vi "4Pi Capture Manager.vi"(7 "Calling VI Ref":refnum<vi>) -> ()   [LabVIEW 2021]
uses:
  4Pi Capture Manager Controls/4Pi Capture Switch Laser.ctl
  4Pi Capture Manager Controls/4Pi Capture Switch Line Scan Modes.ctl
  4Pi Capture Manager Controls/4Pi Capture Line Scan Settings.ctl
  4Pi Capture Manager Controls/DM scan mode.ctl
  4Pi Capture Manager Controls/4Pi Capture Acq Settings.ctl
  <vilib>/Utility/miscctls.llb/LVPointTypeDef.ctl
  4Pi Capture Manager Controls/4Pi Capture Notifier Type.ctl
  4Pi Capture Manager Controls/4Pi Capture Actions.ctl
  4Pi Dual DM Control/4Pi Dual DM - Controls/4Pi Dual DM - Mirror Modes.ctl
  <vilib>/vision/Image Controls.llb/IMAQ Image.ctl
  Hardware Configuration/Hardware Configuration Controls/Device Type.ctl
  4Pi Dual DM Control/4Pi Dual DM - Controls/4Pi Dual DM - Standard Action.ctl
  Hardware Configuration/Hardware Configuration Controls/Device Function.ctl
  Device Library/Cameras/Hamamatsu/Orca Flash/Orca Flash Controls/Orca Flash Actions.ctl
  Device Library/Cameras/Hamamatsu/Orca Flash/Orca Flash Controls/Orca Flash Parameters.ctl
  Device Library/Cameras/Hamamatsu/Orca Flash/Orca Flash Controls/Orca Flash Parameter List.ctl
  Device Library/Cameras/Hamamatsu/Orca Flash/Orca Flash Controls/Orca Flash ROI.ctl
  4Pi Capture Manager Controls/4Pi Capture Scan Tracker.ctl
  Device Manager/Common Device Queue/Common Device Controls/Common Device Actions.ctl
  Device Library/Cameras/Hamamatsu/Orca Flash/Orca Flash Controls/Orca Flash Notifier Element.ctl
  Device Library/DAQmx/AO Single Channel Triggered Ramp/AO SCTR Type Defs/AO SCTR Actions.ctl
  Wide Field Drift Correction/WFDC Controls/WFDC External Sync.ctl
  Wide Field Drift Correction/WFDC Controls/WFDC Cycle Pause.ctl
  Wide Field Drift Correction/WFDC Controls/WFDC Status.ctl
  Device Library/Stages/Stages Controls/Stage Actions.ctl
  Device Library/Shutters/Shutter Controls/Shutter Actions.ctl
  Device Library/AOTFs/AOTF Controls/AOTF Actions.ctl
  Device Library/Cameras/Camera Controls/Camera IMAQ Key Info.ctl
  <vilib>/Utility/file.llb/Read Delimited Spreadsheet (DBL).vi
  <vilib>/Utility/file.llb/Write Delimited Spreadsheet (DBL).vi
  shell32.dll
panel:
  in  "Main Tab":T1(tab)
  in  "Sampling Time (s)":dbl min=0.0 format="%#_2f"
  out "Frame":u32(slide) scale=0.0..10.0
  out "Cycle":sgl(slide) scale=0.0..1.0
  in  "Base Save Path":path
  in  "Capture":bool
  in  "Live Preview":bool
  out "Z Step":sgl(slide) scale=0.0..1.0
  in  "File Name":string="Test Image"
  in  "Preview Exposure Time (s)":dbl=0.1 caption="Exposure Time (s)"
  in  "Capture Exposure Time (s)":dbl=0.1 caption="Exposure Time (s)"
  in  "No. of Frames":u32=1 min=1
  in  "No. of Cycles":u16=1 min=1
  in  "No. of Z Steps":u16=1 min=1
  in  "Z Step Size (µm)":dbl min=-10.0 max=10.0
  in  "Switch Laser At":T2=enum."Each Cycle"
  out "Current Cycle":u16
  out "Current Step":u16
  out "Current Frame":u32
  in  "Auto Update Subfolder":bool=TRUE
  in  "Subfolder Name":string="Area"
  in  "Current Laser":u16(ring) items=["560", "642", "405", "488", "940"]
  in  "Save As Preset":bool
  in  "Line Scan Active":bool
  in  "Number of Lines":u32=8 min=1 max=200 step=1
  in  "Line Scan Mode":T3
  in  "Line Scanning Presets":u16(ring) items=["01 FPS", "02 FPS", "04 FPS", "08 FPS", "16 FPS", "40 FPS"]
  in  "Line Scan Settings":T4
  in  "Active option":enum32{"option 1", "option 2", "option 3"}(radio)
  in  "bead collection":bool
  in  "Soft trigger":bool
  in  "DM first":bool
  in  "Amp magnitude":dbl
  in  "DM scan mode":T5 items=["Idle", "Orthogonal", "Random"]
  in  "Amp step size":dbl
  in  "No. Amp steps":u16=1 min=1
  in  "Mirror Mode":u16[](array[numeric])=[1] min=1 max=140
  in  "Camera Settings":bool
  in  "Quadrants On/Off":bool
  in  "Auto Shutter":bool
  in  "acq settings":T6
  in  "Quit":bool
  # "Live Preview"
  # "Capture"
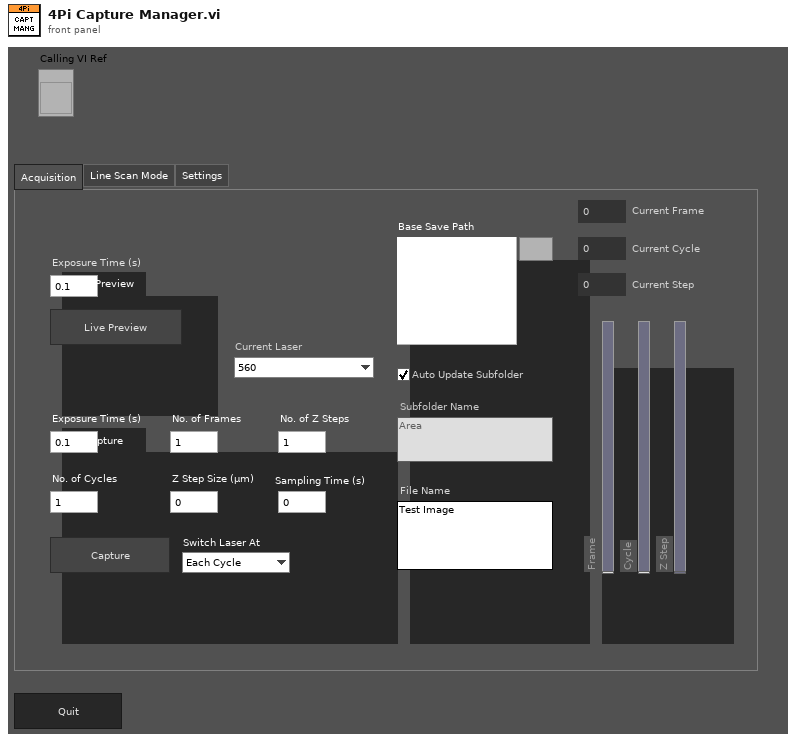
[diagram p1: front panel]
types:
  T1 = enum32{"Acquisition", "Line Scan Mode", "Settings"}
  T2 = typedef "4Pi Capture Switch Laser.ctl" = enum16{"Each Step", "Each Cycle", "All Cycles"}
  T3 = typedef "4Pi Capture Switch Line Scan Modes.ctl" = enum32{"Automatic", "Use Presets", "Manual"}
  T4 = typedef "4Pi Capture Line Scan Settings.ctl" = cluster{"Interline Interval":dbl, "Offset (V)":dbl, "Amplitude (V)":dbl, "Samples Per Channel":dbl, "Delay (ms)":dbl}
  T5 = typedef "DM scan mode.ctl" = u16
  T6 = typedef "4Pi Capture Acq Settings.ctl" = cluster{"Exposure Time (s)":dbl, "No. of Frames":u32, "No. of Z Steps":u16, "No. of Cycles":u16, "Z Step Size (µm)":dbl}
  T7 = typedef "4Pi Dual DM - Standard Action.ctl" = enum16{"Read", "Write"}
  T8 = typedef "IMAQ Image.ctl" = refnum<image>
  T9 = cluster{"Image Ref":T8, "Cycle Number":u16, "Camera Running?":bool, "Capture?":bool}
  T10 = enum8{"Enabled", "Disabled", "Disabled and Grayed Out"}
  T11 = typedef "Device Type.ctl" = enum16{"AOTF", "Camera", "Deformable Mirror", "Laser", "Flip Mirror", "Shutter", "Stage", "Waveform", "FPGA", "Filter Wheel", "Email"}
  T12 = typedef "4Pi Capture Notifier Type.ctl" = cluster{"Actions":T13, "Running?":bool, "Preview Exposure (s)":dbl, "Capture Exposure (s)":dbl, "Cycles":u16, "Frames":u32, "No. of Z Steps":u16, "Z Step Size (µm)":dbl, "Base Path":path, "Init Z Position (µm)":dbl, "Lasers Lines":string[], "Save Path":path, "Line Scan?":bool, "Line Scan Mode":T3, "No. Amp steps":u16, "Amp step size":dbl, "No. Mirror Mode":u16, "DM scan mode":T5, "Metadata File Ref":refnum<file>[], "Init Mirror Modes":T14, "Sampling Time (s)":dbl}
  T13 = typedef "4Pi Capture Actions.ctl" = enum16{"Idle", "Live Preview", "Capture", "Laser On", "Laser Off", "Open Shutters", "Close Shutters", "Set Exposure Time", "Start Acquisition", "Update SubFolder", "Setup", "Camera Soft Trigger", "Camera", "Swtich1", "Switch", "Step", "Cycle", "Write DM", "External Cycle Sync", "Write Metadata", "Abort", "Quit"}
  T14 = typedef "4Pi Dual DM - Mirror Modes.ctl" = cluster{"Mode":string, "Amplitude":dbl}[]
  T15 = enum16{"Always On", "Always Off", "Off While Running"}
  T16 = typedef "LVPointTypeDef.ctl" = cluster{"Horizontal":i16, "Vertical":i16}
  T17 = typedef "Image Type" = u32
  T18 = typedef "Device Function.ctl" = enum16{"Primary", "Secondary", "Overview", "Wide Field Drift Correction", "642 nm Excitation", "560 nm Excitation", "940 nm Excitation", "546 nm Excitation", "488 nm Excitation", "405 nm Excitation", "Objective Drift Correction", "4Pi Focus Lock", "4Pi Objective Lock", "Objective XY", "Objective Z", "Sample XY", "Sample Coarse Z", "Sample Z", "4Pi Lower", "4Pi Upper", "Em Small", "Em Large", "Ex Small", "Ex Large", "Mojo", "Adj Cavity", "Line Scanning", "Alert"}
  T19 = typedef "Orca Flash Parameters.ctl" = cluster{"Value":dbl, "Orca Flash Parameters":T20}
  T20 = typedef "Orca Flash Parameter List.ctl" = u32
  T21 = enum32{"Page Enabled", "Page Disabled", "Page Disabled & Grayed"}
  T22 = typedef "Orca Flash ROI.ctl" = cluster{"H Offset":i32, "V Offset":i32, "H Width":i32, "V Width":i32}
  T23 = typedef "Orca Flash Actions.ctl" = enum16{"IDLE", "PREVIEW", "RECORD", "Send Trigger", "SOFT TRIGGER", "Record Settings", "SETPARAM", "GETPARAM", "SETROI", "GETROI", "PROGRESSIVE MODE", "AREA MODE", "STATUS", "QUIT"}
  T24 = typedef "4Pi Capture Scan Tracker.ctl" = cluster{"Current Step":u16, "Current Cycle":u16, "Current Laser":u16, "# of Lasers":u16, "# of Cycles":u16, "# of Steps":u16, "Switch Laser At":T2, "Current Mirror Mode":u16, "# of Mirror Mode":u16, "Current Amp step":u16, "# of Amp steps":u16}
  T25 = typedef "WFDC Status.ctl" = enum16{"Idle", "Busy", "DC Active", "Error", "Canceled"}
  T26 = typedef "WFDC External Sync.ctl" = cluster{"Cycle Sync":T27, "Z Offset":dbl, "WFDC Status":T25}
  T27 = typedef "WFDC Cycle Pause.ctl" = enum16{"Pause Requested", "Paused", "Resume Requested", "Resumed"}
  T28 = typedef "Stage Actions.ctl" = enum16{"Get Position", "SERVO OFF", "SERVO ON", "SERVO ON/OFF", "MVR", "MOVE", "HALT", "ONTARGET", "ERROR", "REFERENCE", "INIT", "VELOCITY", "STATUS", "EXIT", "HOME", "ZEROPOS", "NANOPOS", "ANALOG", "QUIT"}
  T29 = typedef "Shutter Actions.ctl" = enum16{"Open", "Close", "Toggle", "Status", "Quit"}
  T30 = typedef "AOTF Actions.ctl" = enum16{"Error Check", "Blank", "Line On/Off", "Set Power", "Status", "Quit"}
  T31 = typedef "AO SCTR Actions.ctl" = enum16{"Stop at Offset", "Update and Run", "Quit"}
  T32 = enum16{"open", "replace", "create", "open or create", "replace or create", "replace or create with confirmation"}
  T33 = typedef "Camera IMAQ Key Info.ctl" = cluster{"Frame":u32, "Sensor Height":i32, "Sensor Width":i32, "ROI Height":i32, "ROI Width":i32, "ROI Enable?":bool, "Bit per Pixel":u8}
  T34 = typedef "Orca Flash Notifier Element.ctl" = cluster{"Camera Actions":T23, "Received?":bool, "Running?":bool, "sCMOS Parameter":T19, "sCMOS ROI":T22, "Save Path":path, "# of frames":u32, "Image Ref":T8, "Trigger?":bool, "bead collection":bool}
  T35 = typedef "Common Device Actions.ctl" = enum16{"Specific Action", "Open Front Panel", "Close Front Panel", "Quit", "Quit All"}
  T36 = typedef "4Pi Dual DM - Mirror Modes DUAL.ctl" = cluster{"Mode":string, "Amplitude":dbl}[][]
  T37 = typedef "LVRectTypeDef.ctl" = cluster{"Left":i16, "Top":i16, "Right":i16, "Bottom":i16}
  T38 = typedef "LVBoundsTypeDef.ctl" = cluster{"Width":u32, "Height":u32}
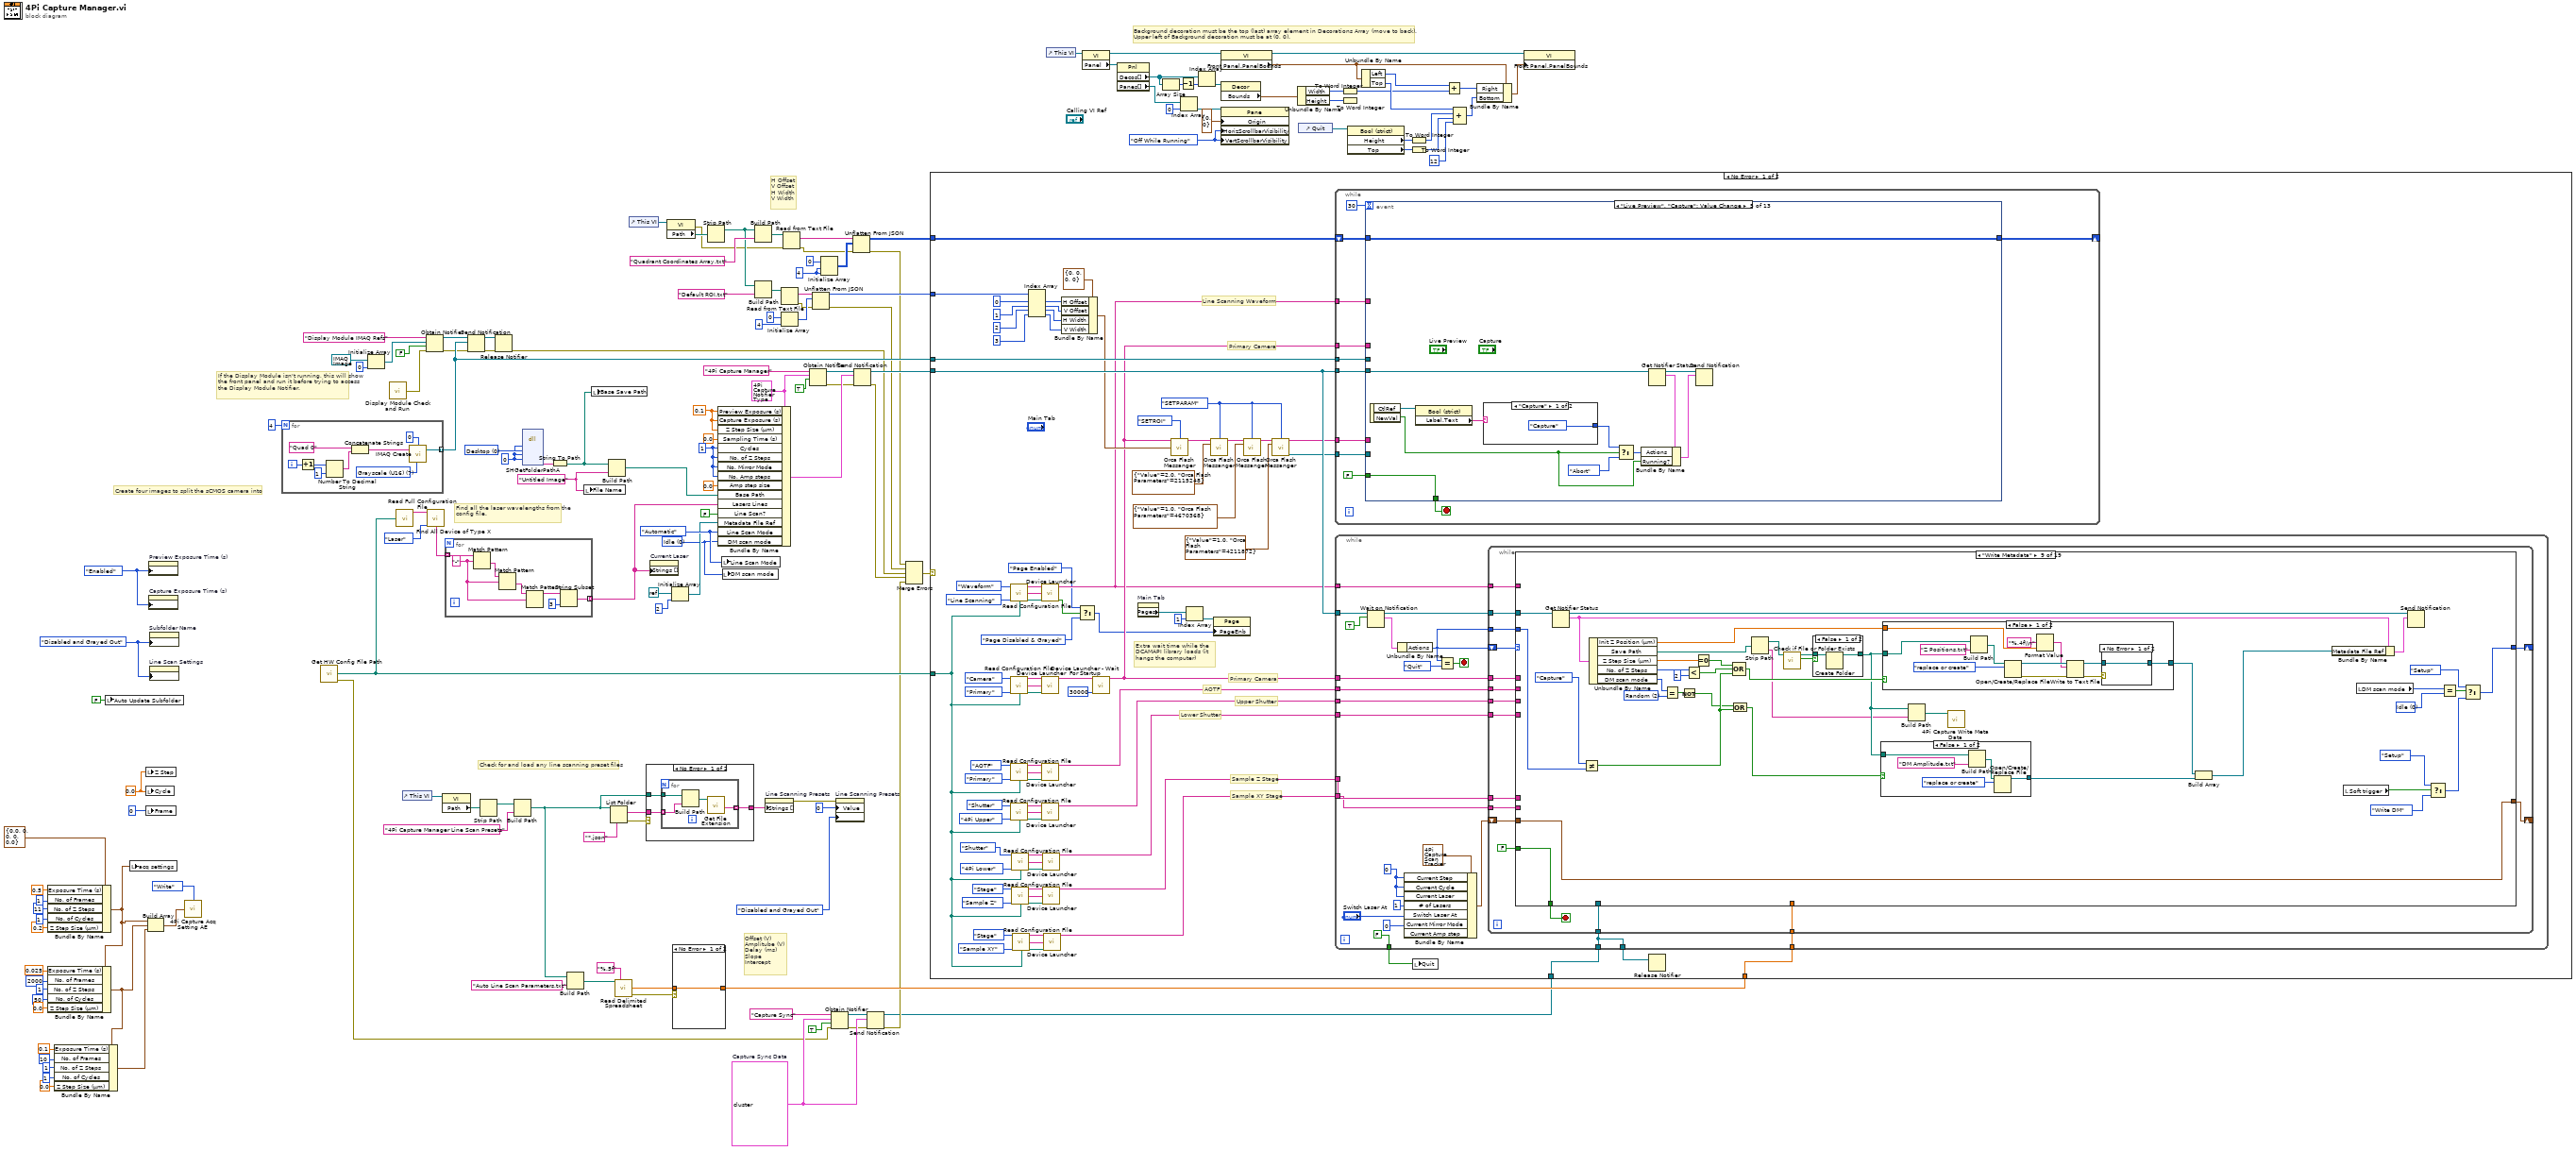
[diagram p0: block diagram]
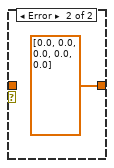
[diagram p2: hidden frame]
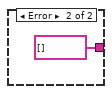
[diagram p3: hidden frame]
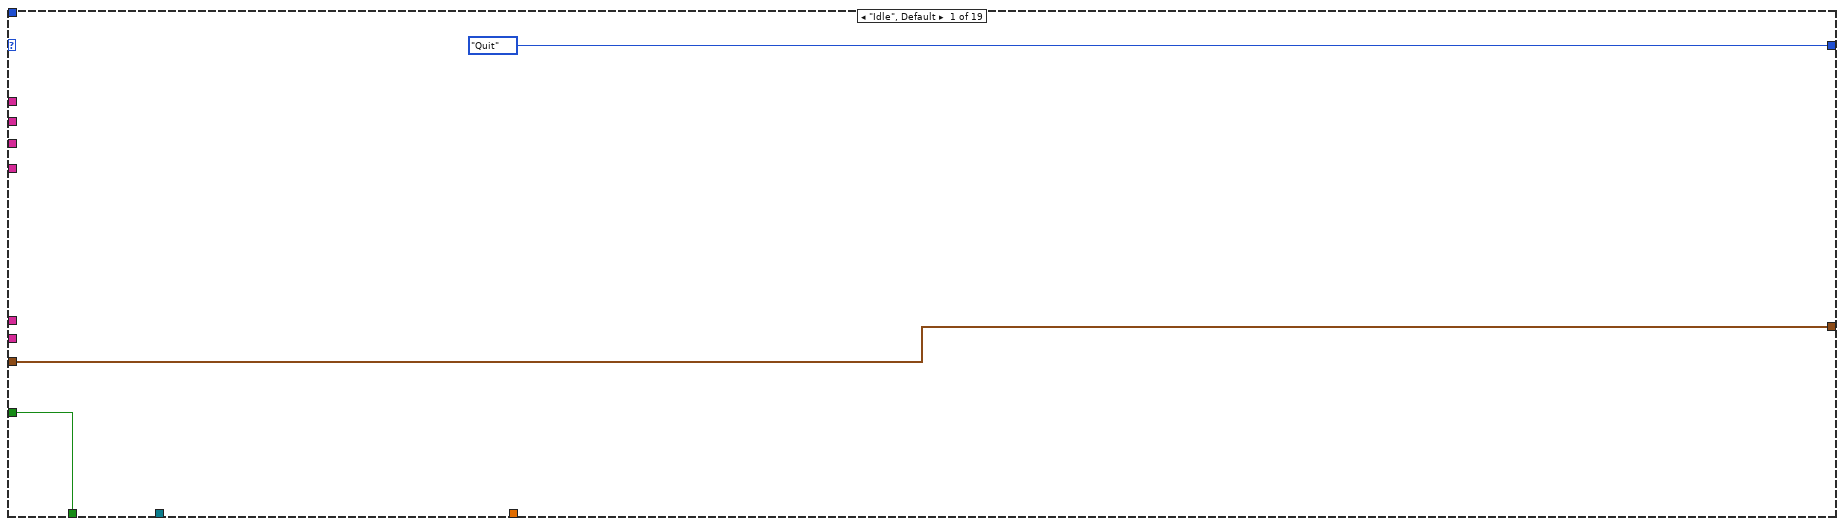
[diagram p4: hidden frame]
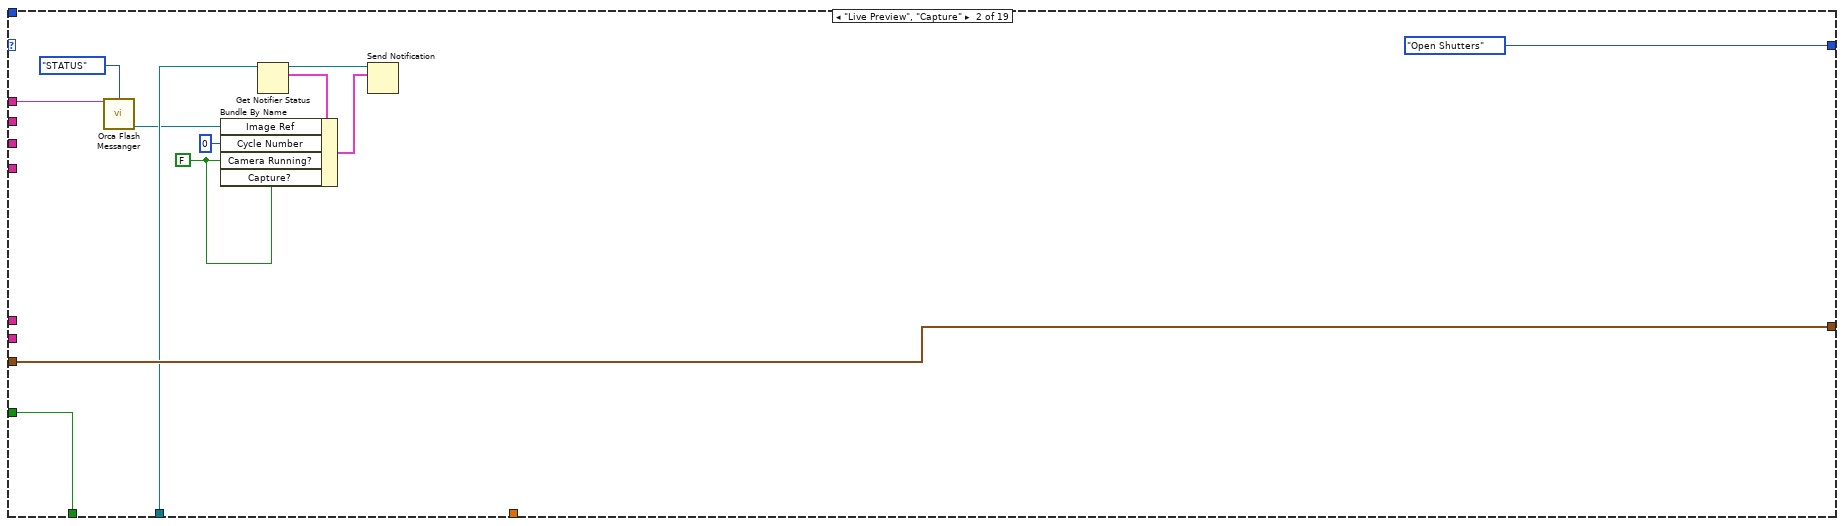
[diagram p5: hidden frame]
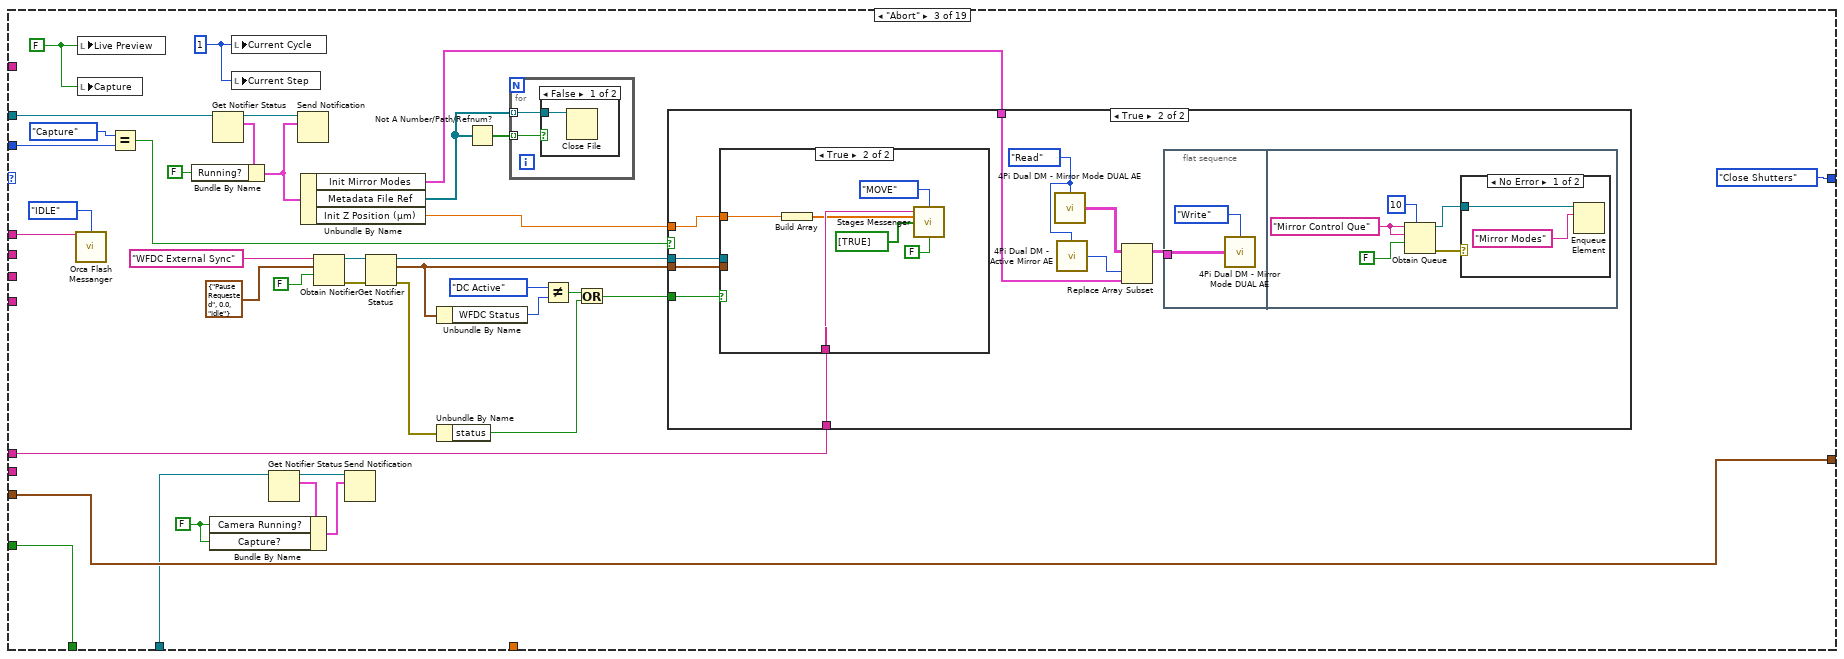
[diagram p6: hidden frame]
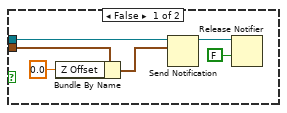
[diagram p10: hidden frame]
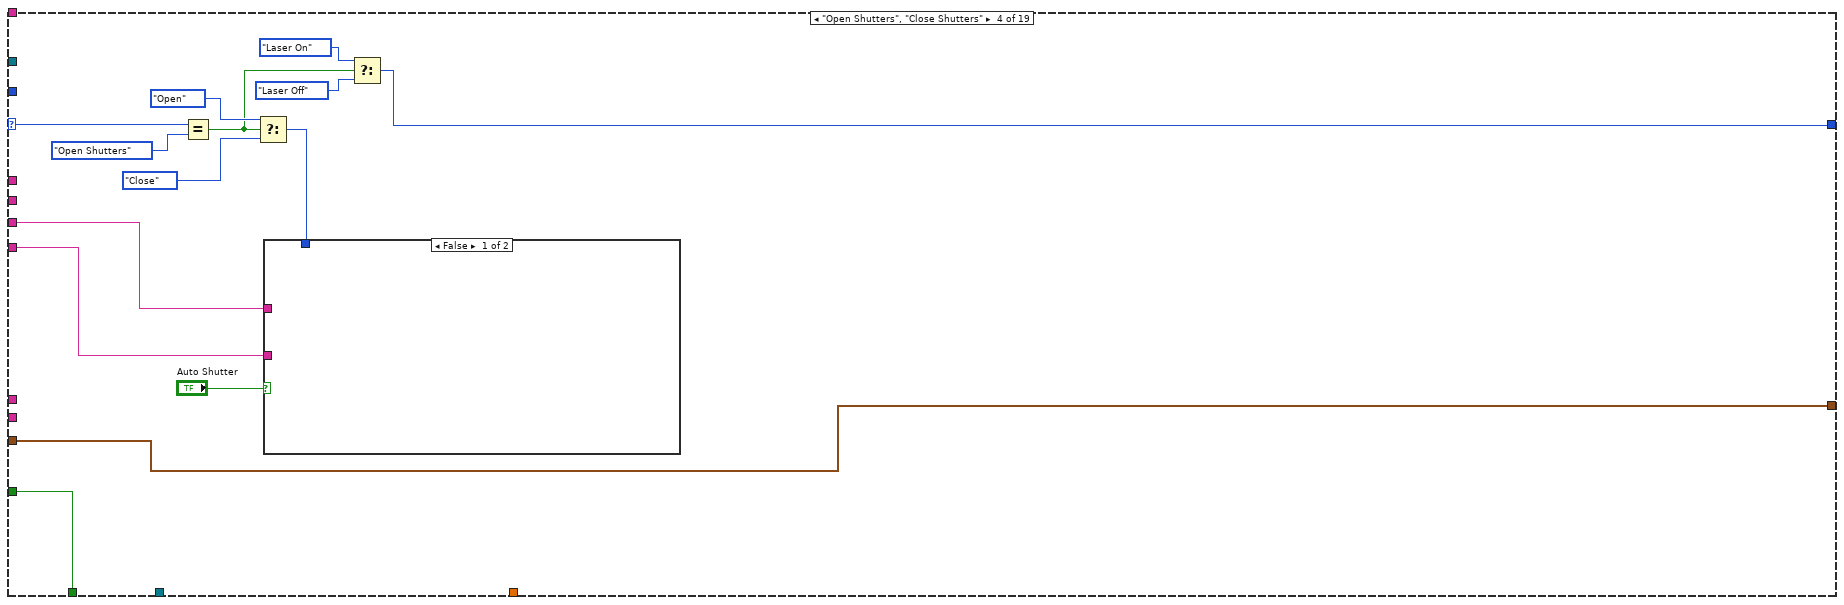
[diagram p11: hidden frame]
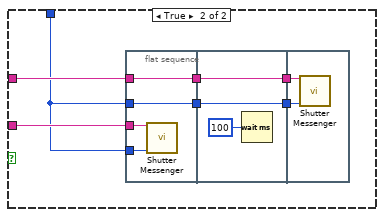
[diagram p12: hidden frame]
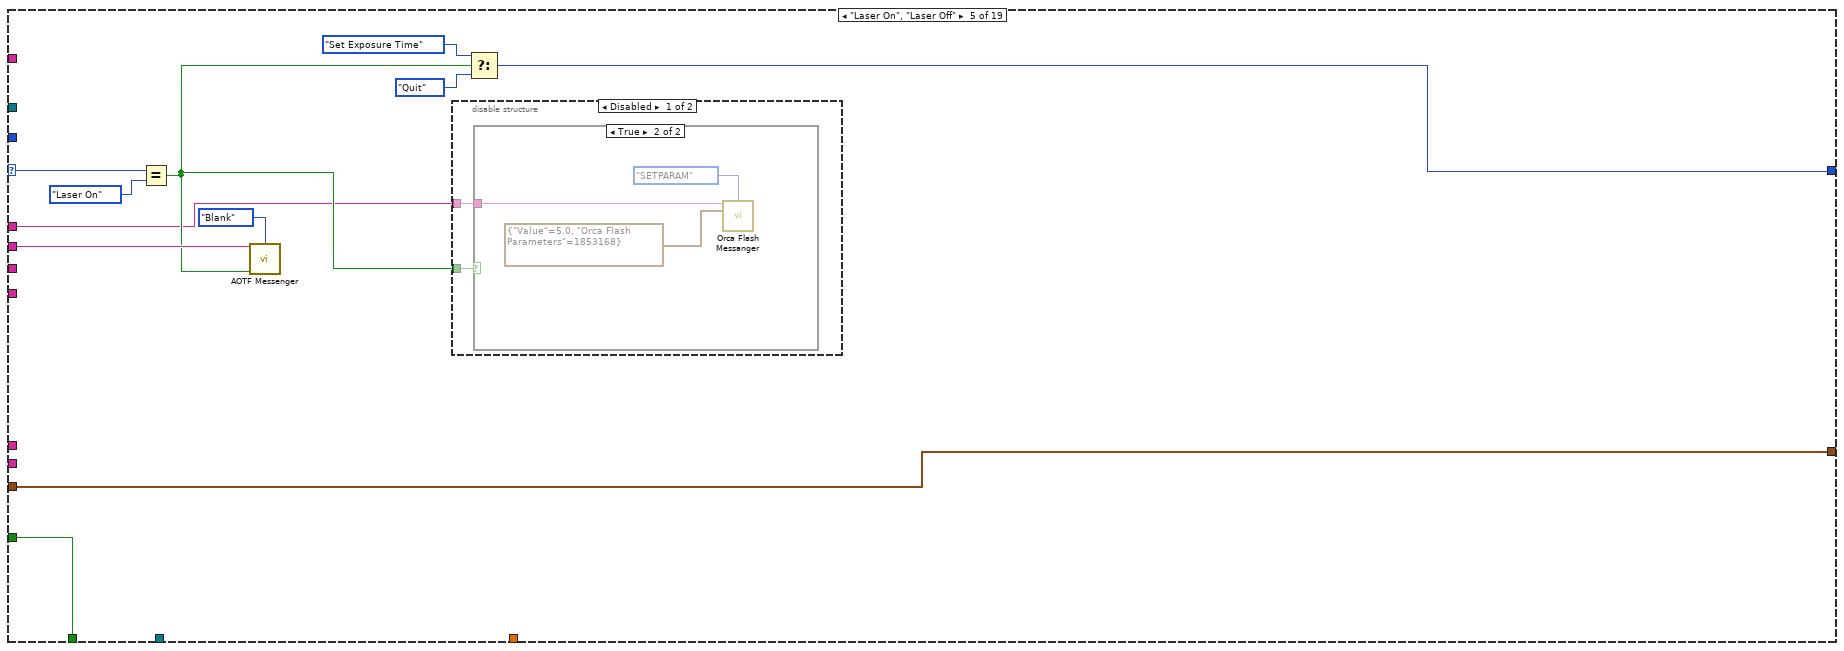
[diagram p13: hidden frame]
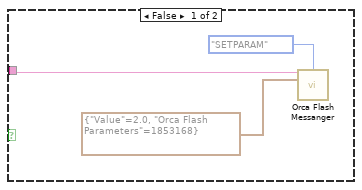
[diagram p14: hidden frame]
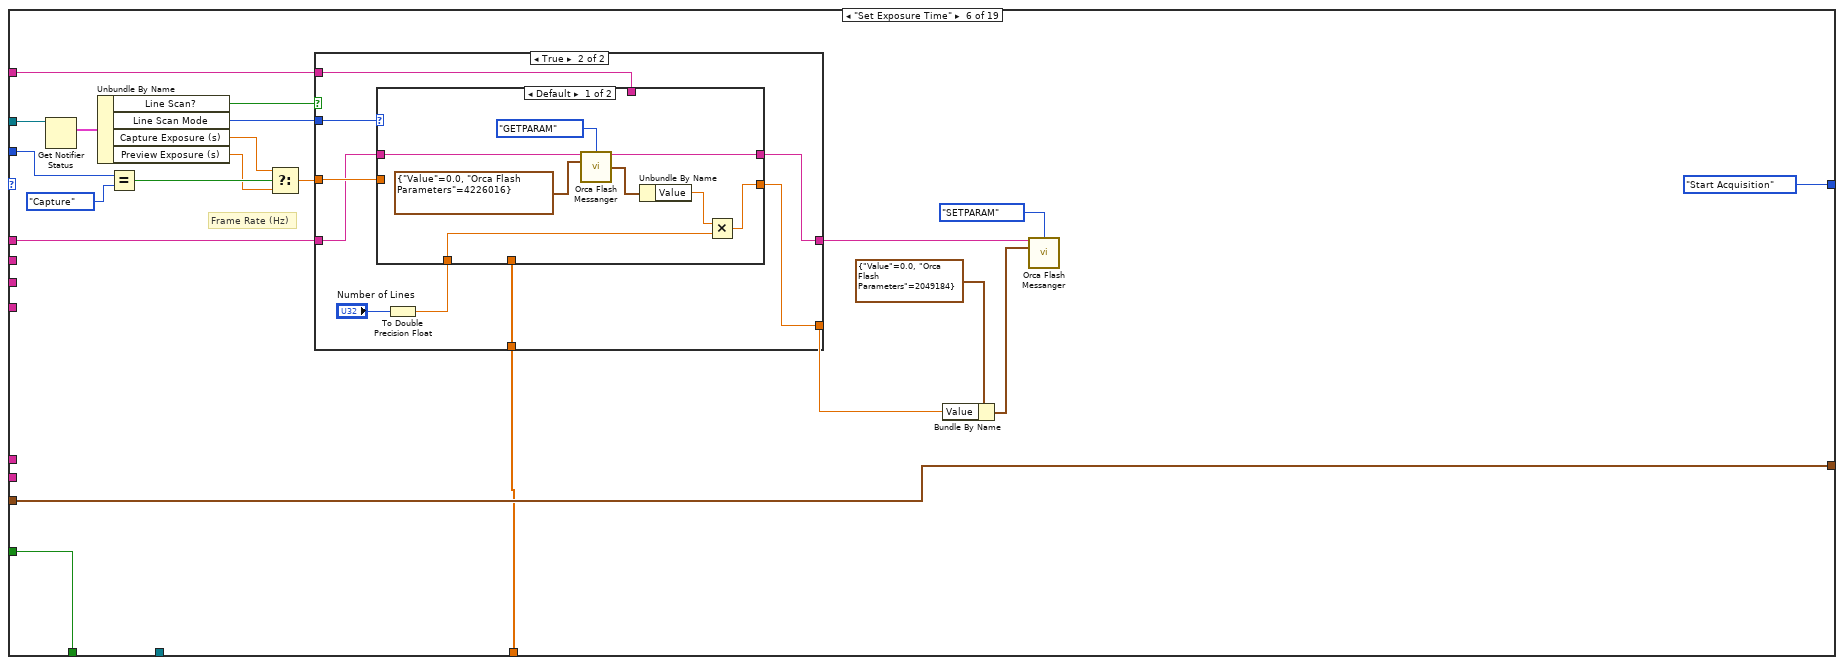
[diagram p16: hidden frame]
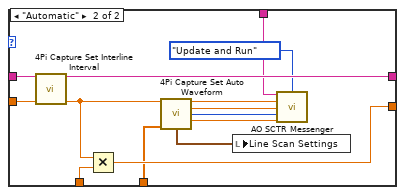
[diagram p18: hidden frame]
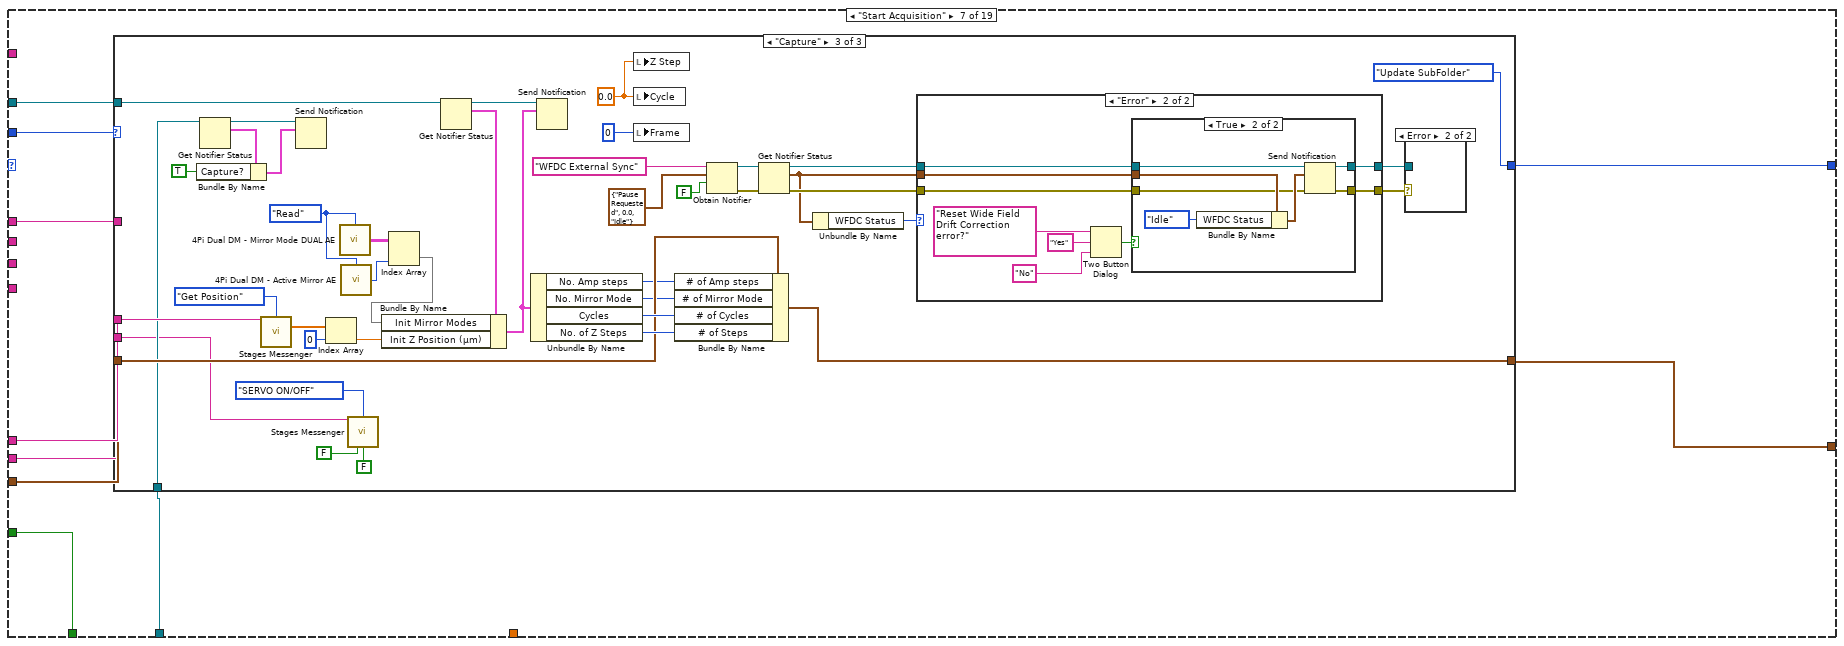
[diagram p19: hidden frame]
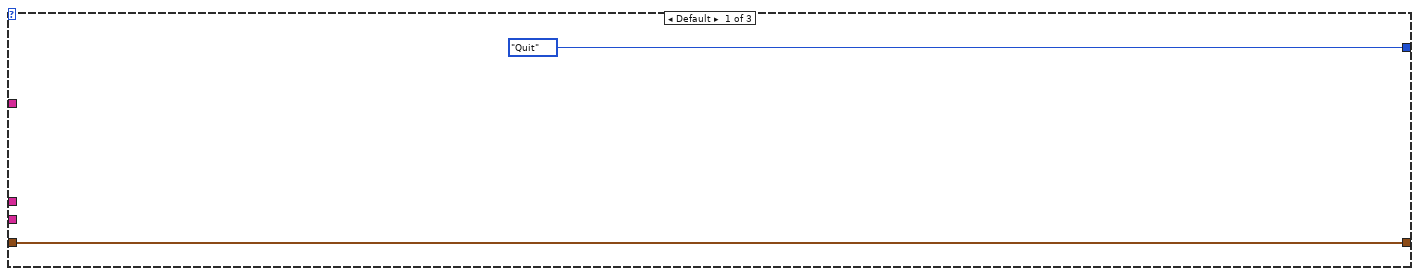
[diagram p20: hidden frame]
diagram:
  w26 = T5 0 items=["Idle", "Orthogonal", "Random"] ("DM scan mode")
  w36 = sgl 0.0 ("Cycle")
  w37 = T9 {"Image Ref"=refnum, "Cycle Number"=0, "Camera Running?"=FALSE, "Capture?"=FALSE}  # Capture Sync Data
  w49 = T10."Enabled" ("Disabled")
  w30 = 4Pi_Capture_Switch_Line_Scan_Modes."Automatic" ("Line Scan Mode")
  w50 = T10."Disabled and Grayed Out" ("Disabled")
  w97 = 4 ("dimension size")
  w101 = "Untitled Image"
  w104 = 0 items=["Desktop"=0, "Personal Documents"=5, "AppData"=26, "Local AppData"=28, "Common AppData"=35, "Program Files"=38, "Program Files Common"=43, "Common Documents"=46] ("Requested Path")
  w103 = 0 ("HWND")
  w25 = u16 1 ("Cycles")
  w24 = 0.1 ("Preview Exposure (s)")
  w107 = T12 {"Actions"=enum."Live Preview", "Running?"=FALSE, "Preview Exposure (s)"=0.1, "Capture Exposure (s)"=0.1, "Cycles"=1, "Frames"=0, "No. of Z Steps"=0, "Z Step Size (µm)"=0.0, "Base Path"=path "", "Init Z Position (µm)"=0.0, "Lasers Lines"=[], "Save Path"=path "", "Line Scan?"=FALSE, "Line Scan Mode"=enum."Automatic", "No. Amp steps"=0, "Amp step size"=0.0, "No. Mirror Mode"=0, "DM scan mode"=0, "Metadata File Ref"=[], "Init Mirror Modes"=[], "Sampling Time (s)"=0.0} ("4Pi Capture Notifier Type")
  w129 = T15."Off While Running" ("Vertical Scrollbar Visibility")
  # "Offset (V)\nAmplitube (V)\nDelay (ms)\nSlope\nIntercept"
  # "Check for and load any line scanning preset files"
  # "Find all the laser wavelengths from the config file."
  # "If the Display Module isn't running, this will show the front panel and run it before trying to access the Display Module Notifier."
  # "H Offset\nV Offset\nH Width\nV Width"
  # "Create four images to split the sCMOS camera into"
  # "Background decoration must be the top (last) array element in Decorations Array (move to back).\nUpper left of Background decoration must be at (0, 0)."
  n1 = Bundle By Name(cluster=T6 {"Exposure Time (s)"=0.0, "No. of Frames"=0, "No. of Z Steps"=0, "No. of Cycles"=0, "Z Step Size (µm)"=0.0} ("acq settings"), "Exposure Time (s)"=0.5, "No. of Frames"=u32 1, "No. of Z Steps"=u16 11, "No. of Cycles"=u16 1, "Z Step Size (µm)"=0.2) -> (w1:T6)
  n2 = Bundle By Name(cluster=w1, "Exposure Time (s)"=0.025, "No. of Frames"=u32 2000, "No. of Z Steps"=u16 1, "No. of Cycles"=u16 50, "Z Step Size (µm)"=0.0) -> (w4:T6)
  n3 = Bundle By Name(cluster=w4, "Exposure Time (s)"=0.1, "No. of Frames"=u32 10, "No. of Z Steps"=u16 1, "No. of Cycles"=u16 1, "Z Step Size (µm)"=0.0) -> (w3:T6)
  n4 = local write "Auto Update Subfolder"(FALSE ("Auto Update Subfolder")) -> ()
  n5 = local write "acq settings"(w1) -> ()
  n6 = local write "Z Step"(w36) -> ()
  n7 = local write "Cycle"(w36) -> ()
  n8 = local write "Frame"(u32 0 ("Frame")) -> ()
  n9 = Build Array(w1, w4, w3) -> (w2:T6[])
  n10 = property on="Preview Exposure Time (s)" class="DigNum (strict)"("DisabledEnum"=w49) -> ()  [unwired: 2 in, 2 out]
  n11 = property on="Capture Exposure Time (s)" class="DigNum (strict)"("DisabledEnum"=w49) -> ()  [unwired: 2 in, 2 out]
  n12 = property on="Subfolder Name" class="Str"("DisabledEnum"=w50) -> ()  [unwired: 2 in, 2 out]
  n13 = property on="Line Scan Settings" class="Clust (strict)"("DisabledEnum"=w50) -> ()  [unwired: 2 in, 2 out]
  n14 = call "4Pi Capture Acq Setting AE.vi"("Action"=4Pi_Dual_DM_-_Standard_Action."Write", "Acq Setting in"=w2) -> ()  [unwired: 13 in, 1 out]
  n15 = for {
    N: 4 -> [_]
    tunnel: [w147] -> w111 mode=indexing
    i -> [w155]
    w150 = T17 7 items=["Grayscale (U8)", "Grayscale (I16)", "Grayscale (SGL)", "Complex (CSG)", "RGB (U32)", "HSL (U32)", "RGB (U64)", "Grayscale (U16)"] ("Image Type")
    n16 = Increment(x=w155) -> (x+1=w153:i32)
    n17 = Number To Decimal String(number=w153, width (-)=i16 1) -> (decimal integer string=w151:string)
    n18 = Concatenate Strings("Quad 0" ("name (unnamed)"), w151) -> (w148:string)
    n19 = call "IMAQ Create"("Border Size"=0, "Image Name"=w148, "Image Type"=w150) -> ("New Image"=w147:T8)  [unwired: 2 in, 1 out]
  }
  n20 = call "Get HW Config File Path.vi"() -> ("File Path"=w64:path, "Error"=w34:errorcluster)  [unwired: 14 in]
  n21 = Initialize Array(T8 refnum ("New Image"), 0 ("dimension size")) -> (w69:T8[])
  n22 = call "Display Module Check and Run.vi"() -> ("Error"=w68:errorcluster)  [unwired: 15 in]
  n23 = call "Read Full Configuration File.vi"("Config File Path"=w64) -> ("Unique Notifier Names"=w65:string[])  [unwired: 11 in, 3 out]
  n24 = control-ref of="This VI"() -> (w61:refnum<vi>)
  n25 = Obtain Notifier(name (unnamed)="Display Module IMAQ Refs", notification data type=w69, create if not found? (T)=FALSE, error in (no error)=w68) -> (notifier out=w112:refnum<notifier>, error out=w79:errorcluster)  [unwired: 1 out]
  n26 = call "Find All Device of Type X.vi"("Unique Notifier Names"=w65, "Device Type"=Device_Type."Laser") -> ("All Devices"=w67:string[])  [unwired: 12 in, 1 out]
  n27 = property class="VI"(reference=w61) -> ("Path"=w60:path)  [unwired: 1 in, 2 out]
  n28 = for {
    tunnel: w67 -> [w157] mode=indexing
    tunnel: [w156] -> w41 mode=indexing
    w160 = "-" ("regular expression")
    n29 = Match Pattern(string=w157, regular expression=w160) -> (after substring=w158:string)  [unwired: 1 in, 3 out]
    n30 = Match Pattern(string=w158, regular expression=w160) -> (after substring=w159:string)  [unwired: 1 in, 3 out]
    n31 = Match Pattern(string=w159, regular expression=w160) -> (before substring=w161:string)  [unwired: 1 in, 3 out]
    n32 = String Subset(string=w161, length (rest)=3 ("length (rest)")) -> (substring=w156:string)  [unwired: 1 in]
  }
  n33 = Send Notification(notification=w111, notifier=w112, error in (no error)=w79) -> (notifier out=w99:refnum<notifier>, error out=w84:errorcluster)
  n34 = Strip Path(path=w60) -> (stripped path=w59:path)  [unwired: 1 out]
  n35 = Release Notifier(notifier=w99, error in (no error)=w84) -> (error out=w76:errorcluster)  [unwired: 1 in, 2 out]
  n36 = Build Path(base path=w59, name or relative path="4Pi Capture Manager Line Scan Presets") -> (appended path=w48:path)
  n37 = dll-call lib="shell32.dll" fn="SHGetFolderPathA"("HWND"=w103, "nFolder"=w104, "hToken"=w103, "dwFlags"=w103) -> ("pszPath"=w102:string)  [unwired: 9 in, 2 out]
  n38 = String To Path(string=w102) -> (path=w100:path)
  n39 = Build Path(base path=w48, name or relative path="Auto Line Scan Parameters.txt") -> (appended path=w46:path)
  n40 = local write "File Name"(w101) -> ()
  n41 = local write "Base Save Path"(w100) -> ()
  n42 = Build Path(base path=w100, name or relative path=w101) -> (appended path=w105:path)
  n43 = List Folder(path=w48, pattern="*.json") -> (filenames=w56:string[], error out=w55:errorcluster)  [unwired: 2 in, 2 out]
  n44 = call-poly <vilib>:"Read Delimited Spreadsheet.vi"("file path (dialog if empty)"=w46, "format (%.3f)"="%.5f") -> ("first row"=w43:dbl[], "error out"=w44:errorcluster)  [unwired: 8 in, 4 out]
  n45 = control-ref of="This VI"() -> (w110:refnum<vi>)
  n46 = case shown="No Error" w55 {
    tunnel: w56 -> [w165 _]
    tunnel: w48 -> [w164 _]
    tunnel: [w163 string[] []] -> w54
    frame No Error {
      n47 = for {
        tunnel: w165 -> [w168] mode=indexing
        tunnel: w164 -> [w169]
        tunnel: [w166] -> w163 mode=indexing
        n48 = Build Path(base path=w169, name or relative path=w168) -> (appended path=w167:path)
        n49 = call <vilib>:"Get File Extension.vi"("file"=w167) -> ("filename without extension"=w166:string)  [unwired: 6 in, 4 out]
      }
    }
    frame Error {
    }
  }
  n50 = property on="Current Laser" class="Ring (strict)"("Strings []"=w41) -> ()  [unwired: 2 in, 2 out]
  n51 = property class="VI"(reference=w110) -> (error out=w81:errorcluster, "Path"=w109:path)  [unwired: 1 in, 1 out]
  n52 = Initialize Array(refnum<k0> refnum, 2 ("dimension size")) -> (w27:refnum<k0>[])
  n53 = case shown="No Error" w44 {
    tunnel: w43 -> [w171 _]
    tunnel: [w171 dbl[] [0.0, 0.0, 0.0, 0.0, 0.0] ("first row")] -> w42
    frame No Error {
    }
    frame Error {
    }
  }
  n54 = Strip Path(path=w109) -> (stripped path=w92:path)  [unwired: 1 out]
  n55 = Bundle By Name(cluster=w107, "Preview Exposure (s)"=w24, "Capture Exposure (s)"=w24, "Z Step Size (µm)"=w24, "Sampling Time (s)"=0.0, "Cycles"=w25, "No. of Z Steps"=w25, "No. Mirror Mode"=w25, "No. Amp steps"=w25, "Amp step size"=0.0, "Base Path"=w105, "Lasers Lines"=w41, "Line Scan?"=FALSE, "Metadata File Ref"=w27, "Line Scan Mode"=w30, "DM scan mode"=w26) -> (w106:T12)
  n56 = local write "Line Scan Mode"(w30) -> ()
  n57 = local write "DM scan mode"(w26) -> ()
  n58 = Build Path(base path=w92, name or relative path="Quadrant Coordinates Array.txt") -> (appended path=w95:path)
  n59 = Build Path(base path=w92, name or relative path="Default ROI.txt") -> (appended path=w90:path)
  n60 = property on="Line Scanning Presets" class="Ring (strict)"("Strings []"=w54) -> (error out=w53:errorcluster)  [unwired: 2 in, 1 out]
  n61 = Read from Text File(file (use dialog)=w90) -> (text=w89:string, error out=w82:errorcluster)  [unwired: 3 in, 2 out]
  n62 = Initialize Array(0 ("element"), 4 ("dimension size")) -> (w86:i32[])
  n63 = Read from Text File(file (use dialog)=w95, error in=w81) -> (text=w94:string, error out=w80:errorcluster)  [unwired: 2 in, 2 out]
  n64 = Obtain Notifier(name (unnamed)="4Pi Capture Manager", notification data type=w107, create if not found? (T)=TRUE) -> (notifier out=w115:refnum<notifier>, error out=w83:errorcluster)  [unwired: 1 in, 1 out]
  n65 = Unflatten From JSON(JSON string=w89, type and defaults=w86, error in (no error)=w82) -> (value=w85:i32[], error out=w75:errorcluster)  [unwired: 4 in]
  n66 = Initialize Array(0 ("element"), w97, w97) -> (w96:i32[][])
  n67 = Obtain Notifier(name (unnamed)="Capture Sync", notification data type=w37, create if not found? (T)=TRUE, error in (no error)=w34) -> (notifier out=w38:refnum<notifier>, error out=w33:errorcluster)  [unwired: 1 out]
  n68 = property on="Line Scanning Presets" class="Ring (strict)"(error in=w53, "Value"=u16 0, "DisabledEnum"=T10."Disabled and Grayed Out" ("Disabled")) -> ()  [unwired: 1 in, 2 out]
  n69 = Unflatten From JSON(JSON string=w94, type and defaults=w96, error in (no error)=w80) -> (value=w93:i32[][], error out=w74:errorcluster)  [unwired: 4 in]
  n70 = Send Notification(notification=w106, notifier=w115, error in (no error)=w83) -> (notifier out=w114:refnum<notifier>, error out=w77:errorcluster)
  n71 = Send Notification(notification=w37, notifier=w38, error in (no error)=w33) -> (notifier out=w31:refnum<notifier>, error out=w32:errorcluster)
  n72 = Merge Errors(w74, w75, w76, w77, w32) -> (w78:errorcluster)
  n73 = case shown="No Error" w78 {
    tunnel: w64 -> [w174 _]
    tunnel: w114 -> [w232 w1624]
    tunnel: w111 -> [w220 w1622]
    tunnel: w93 -> [w219 _]
    tunnel: w85 -> [w213 _]
    tunnel: w42 -> [w194 _]
    tunnel: w31 -> [w186 _]
    frame No Error {
      w180 = Orca_Flash_Actions."SETPARAM" ("Camera Actions")
      # "Sample XY Stage"
      # "Line Scanning Waveform"
      # "Primary Camera"
      # "Extra wait time while the DCAMAPI library loads (it hangs the computer)"
      # "Sample Z Stage"
      # "Lower Shutter"
      # "Upper Shutter"
      # "AOTF"
      # "Primary Camera"
      n74 = call "Read Configuration File.vi"("Device Type"=Device_Type."Waveform", "Device Function"=Device_Function."Line Scanning", "Config File Path"=w174) -> ("Unique Notifier Name"=w198:string, "Device Ports/IDs/Channels"=w199:string[], "Device Engine Path"=w196:path)  [unwired: 9 in, 1 out]
      n75 = call "Read Configuration File.vi"("Device Type"=Device_Type."Camera", "Device Function"=Device_Function."Primary", "Config File Path"=w174) -> ("Unique Notifier Name"=w252:string, "Device Ports/IDs/Channels"=w251:string[], "Device Engine Path"=w250:path)  [unwired: 9 in, 1 out]
      n76 = call "Read Configuration File.vi"("Device Type"=Device_Type."AOTF", "Device Function"=Device_Function."Primary", "Config File Path"=w174) -> ("Unique Notifier Name"=w243:string, "Device Ports/IDs/Channels"=w244:string[], "Device Engine Path"=w245:path)  [unwired: 9 in, 1 out]
      n77 = call "Read Configuration File.vi"("Device Type"=Device_Type."Shutter", "Device Function"=Device_Function."4Pi Upper", "Config File Path"=w174) -> ("Unique Notifier Name"=w233:string, "Device Ports/IDs/Channels"=w242:string[], "Device Engine Path"=w241:path)  [unwired: 9 in, 1 out]
      n78 = call "Read Configuration File.vi"("Device Type"=Device_Type."Shutter", "Device Function"=Device_Function."4Pi Lower", "Config File Path"=w174) -> ("Unique Notifier Name"=w234:string, "Device Ports/IDs/Channels"=w237:string[], "Device Engine Path"=w238:path)  [unwired: 9 in, 1 out]
      n79 = call "Read Configuration File.vi"("Device Type"=Device_Type."Stage", "Device Function"=Device_Function."Sample Z", "Config File Path"=w174) -> ("Unique Notifier Name"=w227:string, "Device Ports/IDs/Channels"=w225:string[], "Device Engine Path"=w224:path)  [unwired: 9 in, 1 out]
      n80 = call "Read Configuration File.vi"("Device Type"=Device_Type."Stage", "Device Function"=Device_Function."Sample XY", "Config File Path"=w174) -> ("Unique Notifier Name"=w175:string, "Device Ports/IDs/Channels"=w179:string[], "Device Engine Path"=w178:path)  [unwired: 9 in, 1 out]
      n81 = Index Array(array=w213, index #1=0 ("index"), index #2=1 ("index"), index #3=2 ("index"), index #4=3 ("index")) -> (element #1=w208:i32, element #2=w205:i32, element #3=w206:i32, element #4=w207:i32)
      n82 = call "Device Launcher.vi"("Notifier Name"=w198, "Device Ports/IDs/Channels"=w199, "Device Engine Path"=w196) -> ("Notifier Name"=w195:string, "Running?"=w190:bool)  [unwired: 11 in]
      n83 = call "Device Launcher.vi"("Notifier Name"=w252, "Device Ports/IDs/Channels"=w251, "Device Engine Path"=w250) -> ("Notifier Name"=w202:string)  [unwired: 11 in, 1 out]
      n84 = call "Device Launcher.vi"("Notifier Name"=w243, "Device Ports/IDs/Channels"=w244, "Device Engine Path"=w245) -> ("Notifier Name"=w231:string)  [unwired: 11 in, 1 out]
      n85 = call "Device Launcher.vi"("Notifier Name"=w233, "Device Ports/IDs/Channels"=w242, "Device Engine Path"=w241) -> ("Notifier Name"=w230:string)  [unwired: 11 in, 1 out]
      n86 = call "Device Launcher.vi"("Notifier Name"=w234, "Device Ports/IDs/Channels"=w237, "Device Engine Path"=w238) -> ("Notifier Name"=w229:string)  [unwired: 11 in, 1 out]
      n87 = call "Device Launcher.vi"("Notifier Name"=w227, "Device Ports/IDs/Channels"=w225, "Device Engine Path"=w224) -> ("Notifier Name"=w222:string)  [unwired: 11 in, 1 out]
      n88 = call "Device Launcher.vi"("Notifier Name"=w175, "Device Ports/IDs/Channels"=w179, "Device Engine Path"=w178) -> ("Notifier Name"=w173:string)  [unwired: 11 in, 1 out]
      n89 = Bundle By Name(cluster=T22 {"H Offset"=0, "V Offset"=0, "H Width"=0, "V Width"=0} ("Orca Flash ROI"), "H Offset"=w208, "V Offset"=w205, "H Width"=w206, "V Width"=w207) -> (w204:T22)
      n90 = Select(t=T21."Page Enabled" ("Page Enabled State"), s=w190, f=T21."Page Disabled & Grayed" ("Page Enabled State")) -> (s? t:f=w187:T21)
      n91 = call "Device Launcher - Wait For Startup.vi"("Notifier Name"=w202, "Wait Time (ms)"=30000) -> ("Notifier Name (Dup)"=w201:string)  [unwired: 12 in, 1 out]
      n92 = property on="Main Tab" class="TabCtl (strict)"() -> ("Pages"=w193:refnum<vi>[])  [unwired: 2 in, 2 out]
      n93 = call "Orca Flash Messanger.vi"("Notifier Name"=w201, "Camera Actions"=Orca_Flash_Actions."SETROI", "sCMOS ROI"=w204) -> ("Notifier Name Dup"=w218:string)  [unwired: 8 in, 4 out]
      n94 = Index Array(array=w193, index=1) -> (element=w191:refnum<vi>)
      n95 = call "Orca Flash Messanger.vi"("Notifier Name"=w218, "Camera Actions"=w180, "sCMOS Parameter"=T19 {"Value"=2.0, "Orca Flash Parameters"=2115248}) -> ("Notifier Name Dup"=w217:string)  [unwired: 8 in, 4 out]
      n96 = property class="Page"(reference=w191, "PageEnb"=w187) -> ()  [unwired: 1 in, 2 out]
      n97 = call "Orca Flash Messanger.vi"("Notifier Name"=w217, "Camera Actions"=w180, "sCMOS Parameter"=T19 {"Value"=1.0, "Orca Flash Parameters"=4670368}) -> ("Notifier Name Dup"=w184:string)  [unwired: 8 in, 4 out]
      n98 = call "Orca Flash Messanger.vi"("Notifier Name"=w184, "Camera Actions"=w180, "sCMOS Parameter"=T19 {"Value"=1.0, "Orca Flash Parameters"=4211872}) -> ("Notifier Name Dup"=w183:string, "Image Ref"=w182:T8)  [unwired: 8 in, 3 out]
      n99 = while {
        tunnel: w232 -> [w1193]
        tunnel: w183 -> [w1192]
        tunnel: w182 -> [w1190]
        tunnel: w220 -> [w1189]
        shift-right: [w1187] -> _
        shift-left: w219 -> [w1188]
        tunnel: w201 -> [w1186]
        tunnel: w195 -> [w1185]
        stop <- w1195 stop-if-true
        n100 = event shown="[4] \"Live Preview\", \"Capture\": Value Change" {
          selector: _ -> [_ _ _ _ _ _ _ _ _ _ _ _ _]
          dyn-events: _ -> [_ _ _ _ _ _ _ _ _ _ _ _ _]
          timeout: 30 -> [_ _ _ _ _ _ _ _ _ _ _ _ _]
          tunnel: [w1220 w1258 _ _ w1407 w1428 w1484 w1509 w1531 w1547 w1567 w1591 w1620] -> w1195
          tunnel: FALSE -> [w1220 w1258 _ _ w1407 w1428 w1484 w1509 w1531 w1547 w1567 w1591 _]
          tunnel: w1193 -> [w1214 w1255 _ _ w1404 _ _ w1503 w1529 _ w1565 _ w1619]
          tunnel: w1192 -> [_ w1254 _ _ _ _ _ _ _ _ _ _ _]
          tunnel: w1190 -> [w1218 _ _ _ _ w1412 _ _ _ _ _ _ _]
          tunnel: w1189 -> [w1219 _ _ _ _ w1418 _ _ _ _ _ _ w1607]
          tunnel: w1188 -> [w1217 w1253 w1377 w1389 w1396 w1411 w1479 w1486 w1530 w1548 w1566 w1583 w1606]
          tunnel: [w1217 w1253 w1377 w1389 w1396 w1410 w1479 w1486 w1530 w1548 w1566 w1583 w1606] -> w1187
          tunnel: w1186 -> [_ _ _ _ _ _ _ w1497 _ _ w1551 _ _]
          tunnel: w1185 -> [_ _ _ _ _ _ _ w1487 _ _ w1559 _ _]
          event Timeout {
            # "Convert to array and then crop. If you\nextract or mask image the destination\nimage custom data keys are overwritten."
            n101 = event-data() -> ()  [unwired: 1 in, 1 out]
            n102 = call "IMAQ ImageToArray"("Image"=w1218) -> ("Image Pixels (U16)"=w1216:u16[][])  [unwired: 3 in, 4 out]
            n103 = for {
              tunnel: w1219 -> [w1251] mode=indexing
              tunnel: w1216 -> [w1252]
              tunnel: w1217 -> [w1249] mode=indexing
              n104 = Index Array(array=w1249, index #1=0 ("index"), index #2=2 ("index"), index #3=1 ("index"), index #4=3 ("index")) -> (element #1=w1247:i32, element #2=w1246:i32, element #3=w1242:i32, element #4=w1241:i32)
              n105 = Array Subset(array=w1252, index (row)=w1247, length (row)=w1246, index (col)=w1242, length (col)=w1241) -> (w1250:u16[][])
              n106 = call "IMAQ ArrayToImage"("Image Pixels (U16)"=w1250, "Image"=w1251) -> ()  [unwired: 8 in, 2 out]
            }
            n107 = local read "Soft trigger"() -> (w1201:bool)
            n108 = local read "No. Amp steps"() -> (w1200:u16)
            n109 = case shown="True" w1201 {
              tunnel: [w1221 w1222] -> w1197
              tunnel: w1200 -> [_ w1223]
              frame False {
                n110 = local read "No. of Frames"() -> (w1221:u32)
              }
              frame True {
                n111 = To Unsigned Long Integer(number=w1223) -> (unsigned 32bit integer=w1222:u32)
                n112 = local write "No. of Frames"(w1222) -> ()
              }
            }
            n113 = local read "Mirror Mode"() -> (w1209:u16[])
            n114 = local read "Soft trigger"() -> (w1203:bool)
            n115 = local read "DM scan mode"() -> (w1208:T5)
            n116 = local read "No. of Cycles"() -> (w1206:u16)
            n117 = local read "Amp step size"() -> (w1210:dbl)
            n118 = local read "DM first"() -> (w1204:bool)
            n119 = local read "Capture Exposure Time (s)"() -> (w1196:dbl)
            n120 = local read "Z Step Size (µm)"() -> (w1211:dbl)
            n121 = local read "No. of Z Steps"() -> (w1212:u16)
            n122 = Array Size(array=w1209) -> (size(s)=w1207:i32)
            n123 = Or(x=w1204, y=w1203) -> (x .or. y?=w1202:bool)
            n124 = case shown="1" w1208 {
              tunnel: w1207 -> [_ w1228]
              tunnel: w1200 -> [_ w1229]
              tunnel: [w1224 w1227] -> w1205
              tunnel: w1202 -> [_ w1226]
              tunnel: w1206 -> [w1224 w1225]
              frame Default {
              }
              frame 1 {
                n125 = case shown="False" w1226 {
                  tunnel: w1229 -> [w1235 _]
                  tunnel: w1228 -> [w1234 w1240]
                  tunnel: [w1230 w1239] -> w1227
                  tunnel: w1225 -> [_ _]
                  frame False {
                    n126 = To Unsigned Word Integer(number=w1234) -> (unsigned 16bit integer=w1233:u16)
                    n127 = Multiply(x=w1233, y=w1235) -> (x*y=w1231:u16)
                    n128 = Equal To 0?(x=w1231) -> (x = 0?=w1232:bool)
                    n129 = case shown="True" w1232 {
                      tunnel: w1231 -> [w1236 w1238]
                      tunnel: [w1236 w1237] -> w1230
                      frame False {
                      }
                      frame True {
                        n130 = Increment(x=w1238) -> (x+1=w1237:u16)
                      }
                    }
                  }
                  frame True {
                    n131 = To Unsigned Word Integer(number=w1240) -> (unsigned 16bit integer=w1239:u16)
                  }
                }
              }
            }
            n132 = Get Notifier Status(notifier=w1214) -> (notifier out=w1215:refnum<notifier>, current notification=w1198:T12)  [unwired: 1 in, 3 out]
            n133 = Bundle By Name(cluster=w1198, "Actions"=4Pi_Capture_Actions."Idle", "Frames"=w1197, "Capture Exposure (s)"=w1196, "No. of Z Steps"=w1212, "Z Step Size (µm)"=w1211, "No. Amp steps"=w1200, "Amp step size"=w1210, "No. Mirror Mode"=w1207, "DM scan mode"=w1208, "Cycles"=w1205) -> (w1213:T12)
            n134 = Send Notification(notification=w1213, notifier=w1215) -> ()  [unwired: 1 in, 2 out]
            n135 = local write "No. of Cycles"(w1205) -> ()
          }
          event "Camera Settings", "Preview Exposure Time (s)", "Capture Exposure Time (s)", "No. of Cycles", "No. of Frames", "No. of Z Steps", "Z Step Size (µm)", "Base Save Path", "File Name", "Amp step size", "Mirror Mode", "No. Amp steps", "Sampling Time (s)", "bead collection": Value Change {
            n136 = event-data() -> ("CtlRef"=w1257:refnum<vi>)  [unwired: 1 in]
            n137 = property class="Ctl"(reference=w1257) -> ("Label.Text"=w1256:string)  [unwired: 1 in, 2 out]
            n138 = case shown="\"No. Amp steps\"" w1256 {
              tunnel: w1255 -> [_ w1262 w1270 w1276 w1282 w1287 w1293 w1303 w1307 w1334 _ w1350 w1359 w1365 _]
              tunnel: w1254 -> [_ _ _ _ _ _ _ _ _ _ w1342 _ _ _ w1372]
              frame Default {
              }
              frame "No. of Cycles" {
                n139 = Get Notifier Status(notifier=w1262) -> (notifier out=w1261:refnum<notifier>, current notification=w1263:T12)  [unwired: 1 in, 3 out]
                n140 = Bundle By Name(cluster=w1263, "Cycles"="No. of Cycles", "Actions"=4Pi_Capture_Actions."Idle") -> (w1264:T12)
                n141 = Send Notification(notification=w1264, notifier=w1261) -> ()  [unwired: 1 in, 2 out]
              }
              frame "No. of Frames" {
                n142 = To Double Precision Float(number="No. of Frames") -> (double precision float=w1266:dbl)
                n143 = property on="Frame" class="Slide (strict)"("Scale.Maximum"=w1266, "Scale.Minimum"=0.0 ("Scale.Range:Minimum")) -> ()  [unwired: 2 in, 2 out]
                n144 = Get Notifier Status(notifier=w1270) -> (notifier out=w1269:refnum<notifier>, current notification=w1271:T12)  [unwired: 1 in, 3 out]
                n145 = Bundle By Name(cluster=w1271, "Frames"="No. of Frames", "Actions"=4Pi_Capture_Actions."Idle") -> (w1272:T12)
                n146 = Send Notification(notification=w1272, notifier=w1269) -> ()  [unwired: 1 in, 2 out]
              }
              frame "No. of Z Steps" {
                n147 = Get Notifier Status(notifier=w1276) -> (notifier out=w1275:refnum<notifier>, current notification=w1277:T12)  [unwired: 1 in, 3 out]
                n148 = Bundle By Name(cluster=w1277, "No. of Z Steps"="No. of Z Steps", "Actions"=4Pi_Capture_Actions."Idle") -> (w1278:T12)
                n149 = Send Notification(notification=w1278, notifier=w1275) -> ()  [unwired: 1 in, 2 out]
              }
              frame "Z Step Size (µm)" {
                n150 = Get Notifier Status(notifier=w1282) -> (notifier out=w1281:refnum<notifier>, current notification=w1283:T12)  [unwired: 1 in, 3 out]
                n151 = Bundle By Name(cluster=w1283, "Z Step Size (µm)"="Z Step Size (µm)", "Actions"=4Pi_Capture_Actions."Idle") -> (w1284:T12)
                n152 = Send Notification(notification=w1284, notifier=w1281) -> ()  [unwired: 1 in, 2 out]
              }
              frame "No. Amp steps" {
                n153 = Get Notifier Status(notifier=w1287) -> (notifier out=w1289:refnum<notifier>, current notification=w1288:T12)  [unwired: 1 in, 3 out]
                n154 = Bundle By Name(cluster=w1288, "No. Amp steps"="No. Amp steps", "Actions"=4Pi_Capture_Actions."Idle") -> (w1290:T12)
                n155 = Send Notification(notification=w1290, notifier=w1289) -> ()  [unwired: 1 in, 2 out]
              }
              frame "Amp step size" {
                n156 = Get Notifier Status(notifier=w1293) -> (notifier out=w1295:refnum<notifier>, current notification=w1296:T12)  [unwired: 1 in, 3 out]
                n157 = Bundle By Name(cluster=w1296, "Amp step size"="Amp step size", "Actions"=4Pi_Capture_Actions."Idle") -> (w1294:T12)
                n158 = Send Notification(notification=w1294, notifier=w1295) -> ()  [unwired: 1 in, 2 out]
              }
              frame "Mirror Mode" {
                n159 = Array Size(array="Mirror Mode") -> (size(s)=w1301:i32)
                n160 = Get Notifier Status(notifier=w1303) -> (notifier out=w1299:refnum<notifier>, current notification=w1302:T12)  [unwired: 1 in, 3 out]
                n161 = Bundle By Name(cluster=w1302, "No. Mirror Mode"=w1301, "Actions"=4Pi_Capture_Actions."Idle") -> (w1298:T12)
                n162 = Send Notification(notification=w1298, notifier=w1299) -> ()  [unwired: 1 in, 2 out]
              }
              frame "DM scan mode" {
                n163 = local read "No. Amp steps"() -> (w1306:u16)
                n164 = local read "Mirror Mode"() -> (w1305:u16[])
                n165 = case shown="1" "DM scan mode" {
                  selector: "DM scan mode" -> [w1310 w1315]
                  tunnel: w1307 -> [w1311 w1324]
                  tunnel: w1306 -> [_ w1321]
                  tunnel: w1305 -> [_ w1322]
                  frame 0, Default {
                    n166 = Get Notifier Status(notifier=w1311) -> (notifier out=w1313:refnum<notifier>, current notification=w1312:T12)  [unwired: 1 in, 3 out]
                    n167 = Bundle By Name(cluster=w1312, "DM scan mode"=w1310, "Actions"=4Pi_Capture_Actions."Idle") -> (w1309:T12)
                    n168 = Send Notification(notification=w1309, notifier=w1313) -> ()  [unwired: 1 in, 2 out]
                  }
                  frame 1 {
                    n169 = Array Size(array=w1322) -> (size(s)=w1319:i32)
                    n170 = Get Notifier Status(notifier=w1324) -> (notifier out=w1317:refnum<notifier>, current notification=w1323:T12)  [unwired: 1 in, 3 out]
                    n171 = To Unsigned Word Integer(number=w1319) -> (unsigned 16bit integer=w1318:u16)
                    n172 = Multiply(x=w1321, y=w1318) -> (x*y=w1320:u16)
                    n173 = Bundle By Name(cluster=w1323, "Actions"=4Pi_Capture_Actions."Idle", "DM scan mode"=w1315, "Cycles"=w1320) -> (w1316:T12)
                    n174 = local write "No. of Cycles"(w1320) -> ()
                    n175 = Send Notification(notification=w1316, notifier=w1317) -> ()  [unwired: 1 in, 2 out]
                  }
                }
              }
              frame "Base Save Path", "File Name", "Save Path" {
                n176 = Path To String(path="Base Save Path") -> (string=w1329:string)
                n177 = Equal?(x="", y=w1329) -> (x = y?=w1327:bool)
                n178 = case shown="False" w1327 {
                  tunnel: [w1337 w1338] -> w1326
                  tunnel: "Base Save Path" -> [w1337 _]
                  frame False {
                  }
                  frame True {
                    w1341 = 0 items=["Desktop"=0, "Personal Documents"=5, "AppData"=26, "Local AppData"=28, "Common AppData"=35, "Program Files"=38, "Program Files Common"=43, "Common Documents"=46] ("Requested Path")
                    w1340 = 0 ("HWND")
                    n179 = dll-call lib="shell32.dll" fn="SHGetFolderPathA"("HWND"=w1340, "nFolder"=w1341, "hToken"=w1340, "dwFlags"=w1340) -> ("pszPath"=w1339:string)  [unwired: 9 in, 2 out]
                    n180 = String To Path(string=w1339) -> (path=w1338:path)
                  }
                }
                n181 = Build Path(base path=w1326, name or relative path="File Name") -> (appended path=w1330:path)
                n182 = Get Notifier Status(notifier=w1334) -> (notifier out=w1333:refnum<notifier>, current notification=w1335:T12)  [unwired: 1 in, 3 out]
                n183 = Bundle By Name(cluster=w1335, "Base Path"=w1330, "Actions"=4Pi_Capture_Actions."Idle") -> (w1336:T12)
                n184 = Send Notification(notification=w1336, notifier=w1333) -> ()  [unwired: 1 in, 2 out]
              }
              frame "Camera Settings" {
                n185 = Select(t=Common_Device_Actions."Open Front Panel" ("Common Actions"), s="Camera Settings", f=Common_Device_Actions."Close Front Panel" ("Common Actions")) -> (s? t:f=w1346:T35)
                n186 = call "Common Device Queue Messenger.vi"("Common Action"=w1346, "Notifier Name"=w1342) -> ()  [unwired: 13 in, 1 out]
              }
              frame "Preview Exposure Time (s)" {
                # "Add in a preview stop\nand restart here"
                n187 = Get Notifier Status(notifier=w1350) -> (notifier out=w1353:refnum<notifier>, current notification=w1352:T12)  [unwired: 1 in, 3 out]
                n188 = Bundle By Name(cluster=w1352, "Preview Exposure (s)"="Preview Exposure Time (s)", "Running?"=FALSE ("Abort"), "Actions"=4Pi_Capture_Actions."Idle") -> (w1351:T12)
                n189 = Send Notification(notification=w1351, notifier=w1353) -> ()  [unwired: 1 in, 2 out]
              }
              frame "Capture Exposure Time (s)" {
                n190 = Get Notifier Status(notifier=w1359) -> (notifier out=w1358:refnum<notifier>, current notification=w1357:T12)  [unwired: 1 in, 3 out]
                n191 = Bundle By Name(cluster=w1357, "Capture Exposure (s)"="Capture Exposure Time (s)", "Actions"=4Pi_Capture_Actions."Idle") -> (w1356:T12)
                n192 = Send Notification(notification=w1356, notifier=w1358) -> ()  [unwired: 1 in, 2 out]
              }
              frame "Sampling Time (s)" {
                n193 = Get Notifier Status(notifier=w1365) -> (notifier out=w1364:refnum<notifier>, current notification=w1363:T12)  [unwired: 1 in, 3 out]
                n194 = Bundle By Name(cluster=w1363, "Sampling Time (s)"="Sampling Time (s)", "Actions"=4Pi_Capture_Actions."Idle") -> (w1362:T12)
                n195 = Send Notification(notification=w1362, notifier=w1364) -> ()  [unwired: 1 in, 2 out]
              }
              frame "bead collection" {
                n196 = Obtain Notifier(name (unnamed)=w1372, notification data type=T34 {"Camera Actions"=enum."IDLE", "Received?"=FALSE, "Running?"=FALSE, "sCMOS Parameter"={"Value"=0.0, "Orca Flash Parameters"=0}, "sCMOS ROI"={"H Offset"=0, "V Offset"=0, "H Width"=0, "V Width"=0}, "Save Path"=path "", "# of frames"=0, "Image Ref"=refnum, "Trigger?"=FALSE, "bead collection"=FALSE} ("Camera Cluster")) -> (notifier out=w1371:refnum<notifier>)  [unwired: 2 in, 2 out]
                n197 = Get Notifier Status(notifier=w1371) -> (notifier out=w1370:refnum<notifier>, current notification=w1369:T34)  [unwired: 1 in, 3 out]
                n198 = Bundle By Name(cluster=w1369, "bead collection"="bead collection") -> (w1367:T34)
                n199 = Send Notification(notification=w1367, notifier=w1370) -> (notifier out=w1366:refnum<notifier>)  [unwired: 1 in, 1 out]
                n200 = Release Notifier(notifier=w1366) -> ()  [unwired: 2 in, 3 out]
              }
            }
          }
          event "Active option": Value Change {
            n201 = event-data() -> ("NewVal"=w1388:enum32{"option 1", "option 2", "option 3"})  [unwired: 1 in]
            n202 = To Long Integer(number=w1388) -> (32bit integer=w1387:i32)
            n203 = call "4Pi Capture Acq Active Option AE.vi"("Action"=4Pi_Dual_DM_-_Standard_Action."Write", "Active Option In"=w1387) -> ("Active Option"=w1383:i32)  [unwired: 13 in]
            n204 = call "4Pi Capture Acq Setting AE.vi"("Action"=4Pi_Dual_DM_-_Standard_Action."Read") -> ("Acq Setting out"=w1384:T6[])  [unwired: 14 in]
            n205 = Index Array(array=w1384, index=w1383) -> (element=w1378:T6)
            n206 = local write "acq settings"(w1378) -> ()
            n207 = Unbundle By Name(w1378) -> ("Exposure Time (s)"=w1382:dbl, "No. of Frames"=w1374:u32, "No. of Z Steps"=w1381:u16, "No. of Cycles"=w1380:u16, "Z Step Size (µm)"=w1379:dbl)
            n208 = local write "Capture Exposure Time (s)"(w1382) -> ()
            n209 = local write "No. of Z Steps"(w1381) -> ()
            n210 = local write "No. of Cycles"(w1380) -> ()
            n211 = local write "Z Step Size (µm)"(w1379) -> ()
            n212 = To Double Precision Float(number=w1374) -> (double precision float=w1376:dbl)
            n213 = local write "No. of Frames"(w1374) -> ()
            n214 = property on="Frame" class="Slide (strict)"("Scale.Maximum"=w1376, "Scale.Minimum"=0.0 ("Scale.Range:Minimum")) -> ()  [unwired: 2 in, 2 out]
          }
          event Value Change {
            w1395 = 4Pi_Dual_DM_-_Standard_Action."Read" ("Action")
            n215 = event-data() -> ()  [unwired: 1 in, 1 out]
            n216 = call "4Pi Capture Acq Active Option AE.vi"("Action"=w1395) -> ("Active Option"=w1393:i32)  [unwired: 14 in]
            n217 = call "4Pi Capture Acq Setting AE.vi"("Action"=w1395) -> ("Acq Setting out"=w1394:T6[])  [unwired: 14 in]
            n218 = Replace Array Subset(array=w1394, new element="acq settings", index=w1393) -> (w1392:T6[])
            n219 = call "4Pi Capture Acq Setting AE.vi"("Action"=4Pi_Dual_DM_-_Standard_Action."Write", "Acq Setting in"=w1392) -> ()  [unwired: 13 in, 1 out]
          }
          event "Live Preview", "Capture": Value Change {
            n220 = event-data() -> ("CtlRef"=w1399:refnum<vi>, "NewVal"=w1402:bool)  [unwired: 1 in]
            n221 = property class="Bool (strict)"(reference=w1399) -> ("Label.Text"=w1398:string)  [unwired: 1 in, 2 out]
            n222 = case shown="\"Capture\"" w1398 {
              tunnel: [4Pi_Capture_Actions."Capture" ("y") 4Pi_Capture_Actions."Live Preview" ("y")] -> w1397
              frame "Capture" {
              }
              frame "Live Preview", Default {
              }
            }
            n223 = Select(t=w1397, s=w1402, f=4Pi_Capture_Actions."Abort" ("y")) -> (s? t:f=w1401:T13)
            n224 = Get Notifier Status(notifier=w1404) -> (notifier out=w1405:refnum<notifier>, current notification=w1403:T12)  [unwired: 1 in, 3 out]
            n225 = Bundle By Name(cluster=w1403, "Actions"=w1401, "Running?"=w1402) -> (w1400:T12)
            n226 = Send Notification(notification=w1400, notifier=w1405) -> ()  [unwired: 1 in, 2 out]
          }
          event "Quadrants On/Off": Value Change {
            n227 = event-data() -> ("NewVal"=w1424:bool)  [unwired: 1 in]
            n228 = Obtain Notifier(name (unnamed)="Display Module IMAQ Refs", notification data type=T8[] [], create if not found? (T)=FALSE) -> (notifier out=w1417:refnum<notifier>, error out=w1416:errorcluster)  [unwired: 1 in, 1 out]
            n229 = Get Notifier Status(notifier=w1417, error in (no error)=w1416) -> (notifier out=w1415:refnum<notifier>, current notification=w1413:T8[], error out=w1414:errorcluster)  [unwired: 2 out]
            n230 = case shown="True" w1424 {
              tunnel: w1415 -> [w1450 w1465]
              tunnel: w1414 -> [w1449 w1464]
              tunnel: [w1446 w1460] -> w1420
              tunnel: [w1450 w1465] -> w1421
              tunnel: [w1449 w1464] -> w1419
              tunnel: w1418 -> [w1441 w1463]
              tunnel: w1413 -> [w1448 w1462]
              tunnel: w1412 -> [w1442 w1459]
              tunnel: w1411 -> [_ w1458]
              tunnel: [w1429 w1458] -> w1410
              frame False {
                w1440 = 4 ("dimension size")
                n231 = control-ref of="This VI"() -> (w1430:refnum<vi>)
                n232 = Equal?(x=w1448, y=w1442) -> (x = y?=w1445:bool[])
                n233 = property class="VI"(reference=w1430) -> (error out=w1438:errorcluster, "Path"=w1431:path)  [unwired: 1 in, 1 out]
                n234 = for {
                  tunnel: w1445 -> [w1457] mode=indexing
                  tunnel: [w1456] -> w1443
                  i -> [w1456]
                  stop <- w1457 stop-if-true
                }
                n235 = Or Array Elements(Boolean array=w1445) -> (logical OR=w1444:bool)
                n236 = Strip Path(path=w1431) -> (stripped path=w1437:path)  [unwired: 1 out]
                n237 = case shown="True" w1444 {
                  tunnel: w1443 -> [_ w1454]
                  tunnel: w1448 -> [w1451 w1453]
                  tunnel: [w1451 w1452] -> w1447
                  frame False {
                  }
                  frame True {
                    n238 = Delete From Array(array=w1453, length=1, index=w1454) -> (array with subset deleted=w1452:T8[])  [unwired: 1 out]
                  }
                }
                n239 = Build Path(base path=w1437, name or relative path="Quadrant Coordinates Array.txt") -> (appended path=w1435:path)
                n240 = Read from Text File(file (use dialog)=w1435, error in=w1438) -> (text=w1436:string, error out=w1439:errorcluster)  [unwired: 2 in, 2 out]
                n241 = Initialize Array(0 ("element"), w1440, w1440) -> (w1434:i32[][])
                n242 = Build Array (concatenate)(w1447, w1441) -> (w1446:T8[])
                n243 = Unflatten From JSON(JSON string=w1436, type and defaults=w1434, error in (no error)=w1439) -> (value=w1429:i32[][])  [unwired: 4 in, 1 out]
              }
              frame True {
                n244 = for {
                  tunnel: w1463 -> [w1468] mode=indexing
                  shift-right: [w1466] -> w1461
                  shift-left: w1462 -> [w1467]
                  n245 = Equal?(x=w1467, y=w1468) -> (x = y?=w1471:bool[])
                  n246 = for {
                    tunnel: w1471 -> [w1478] mode=indexing
                    tunnel: [w1477] -> w1469
                    i -> [w1477]
                    stop <- w1478 stop-if-true
                  }
                  n247 = Or Array Elements(Boolean array=w1471) -> (logical OR=w1470:bool)
                  n248 = case shown="True" w1470 {
                    tunnel: w1469 -> [_ w1475]
                    tunnel: w1467 -> [w1472 w1474]
                    tunnel: [w1472 w1473] -> w1466
                    frame False {
                    }
                    frame True {
                      n249 = Delete From Array(array=w1474, length=1, index=w1475) -> (array with subset deleted=w1473:T8[])  [unwired: 1 out]
                    }
                  }
                }
                n250 = Build Array (concatenate)(w1461, w1459) -> (w1460:T8[])
              }
            }
            n251 = Send Notification(notification=w1420, notifier=w1421, error in (no error)=w1419) -> (notifier out=w1423:refnum<notifier>, error out=w1422:errorcluster)
            n252 = Release Notifier(notifier=w1423, error in (no error)=w1422) -> ()  [unwired: 1 in, 3 out]
          }
          event "Auto Update Subfolder": Value Change {
            n253 = event-data() -> ("NewVal"=w1483:bool)  [unwired: 1 in]
            n254 = Select(t=T10."Enabled" ("Disabled"), s=w1483, f=T10."Disabled and Grayed Out") -> (s? t:f=w1480:T10)
            n255 = property on="Subfolder Name" class="Str"("DisabledEnum"=w1480) -> ()  [unwired: 2 in, 2 out]
          }
          event "Line Scan Active": Value Change {
            n256 = event-data() -> ("NewVal"=w1485:bool)  [unwired: 1 in]
            n257 = Select(t="Frame Rate (Hz)", s=w1485, f="Exposure Time (s)") -> (s? t:f=w1506:string)
            n258 = Select(t=4.0, s=w1485, f=0.1) -> (s? t:f=w1499:dbl)
            n259 = Select(t=-1.0 ("f"), s=w1485, f=0.0) -> (s? t:f=w1490:dbl)
            n260 = Select(t=AO_SCTR_Actions."Update and Run" ("Actions"), s=w1485, f=AO_SCTR_Actions."Stop at Offset" ("Actions")) -> (s? t:f=w1491:T31)
            n261 = property on="Capture Exposure Time (s)" class="DigNum (strict)"("Caption.Text"=w1506, "Value"=w1499) -> ()  [unwired: 2 in, 2 out]
            n262 = property on="Preview Exposure Time (s)" class="DigNum (strict)"("Caption.Text"=w1506, "Value"=w1499) -> ()  [unwired: 2 in, 2 out]
            n263 = call "AO SCTR Messenger.vi"("Notifier Name"=w1487, "Actions"=w1491, "Offset (V)"=w1490) -> ()  [unwired: 12 in, 1 out]
            n264 = case shown="False" w1485 {
              frame False {
                w1510 = T10."Enabled" ("Disabled")
                n265 = property on="Preview Exposure Time (s)" class="DigNum (strict)"("DisabledEnum"=w1510) -> ()  [unwired: 2 in, 2 out]
                n266 = property on="Capture Exposure Time (s)" class="DigNum (strict)"("DisabledEnum"=w1510) -> ()  [unwired: 2 in, 2 out]
              }
              frame True {
              }
            }
            n267 = Get Notifier Status(notifier=w1503) -> (notifier out=w1502:refnum<notifier>, current notification=w1501:T12)  [unwired: 1 in, 3 out]
            n268 = Bundle By Name(cluster=w1501, "Line Scan?"=w1485, "Actions"=4Pi_Capture_Actions."Idle", "Preview Exposure (s)"=w1499, "Capture Exposure (s)"=w1499) -> (w1498:T12)
            n269 = Select(t=Orca_Flash_Actions."PROGRESSIVE MODE" ("Camera Actions"), s=w1485, f=Orca_Flash_Actions."AREA MODE" ("Camera Actions")) -> (s? t:f=w1494:T23)
            n270 = call "Orca Flash Messanger.vi"("Notifier Name"=w1497, "Camera Actions"=w1494) -> ()  [unwired: 9 in, 5 out]
            n271 = Send Notification(notification=w1498, notifier=w1502) -> ()  [unwired: 1 in, 2 out]
          }
          event Value Change {
            n272 = event-data() -> ("NewVal"=w1520:T3)  [unwired: 1 in]
            n273 = Get Notifier Status(notifier=w1529) -> (notifier out=w1528:refnum<notifier>, current notification=w1527:T12)  [unwired: 1 in, 3 out]
            n274 = Bundle By Name(cluster=w1527, "Actions"=4Pi_Capture_Actions."Idle", "Line Scan Mode"=w1520) -> (w1526:T12)
            n275 = Send Notification(notification=w1526, notifier=w1528) -> ()  [unwired: 1 in, 2 out]
            n276 = Equal?(x=w1520, y=4Pi_Capture_Switch_Line_Scan_Modes."Use Presets") -> (x = y?=w1512:bool)
            n277 = Not Equal?(x=w1520, y=4Pi_Capture_Switch_Line_Scan_Modes."Automatic") -> (x != y?=w1514:bool)
            n278 = Select(t=T10."Enabled" ("Disabled"), s=w1512, f=T10."Disabled and Grayed Out" ("Disabled")) -> (s? t:f=w1522:T10)
            n279 = property on="Line Scanning Presets" class="Ring (strict)"("DisabledEnum"=w1522) -> ()  [unwired: 2 in, 2 out]
            n280 = case shown="True" w1512 {
              frame False {
              }
              frame True {
                n281 = property on="Line Scanning Presets" class="Ring (strict)"() -> ("Value"=w1532:u16)  [unwired: 2 in, 2 out]
                n282 = property on="Line Scanning Presets" class="Ring (strict)"("Val(Sgnl)"=w1532) -> ()  [unwired: 2 in, 2 out]
              }
            }
            n283 = Select(t=T10."Disabled and Grayed Out" ("Disabled"), s=w1514, f=T10."Enabled" ("Disabled")) -> (s? t:f=w1513:T10)
            n284 = Select(t=T10."Enabled" ("Disabled"), s=w1514, f=T10."Disabled and Grayed Out" ("Disabled")) -> (s? t:f=w1517:T10)
            n285 = property on="Preview Exposure Time (s)" class="DigNum (strict)"("DisabledEnum"=w1513) -> ()  [unwired: 2 in, 2 out]
            n286 = property on="Capture Exposure Time (s)" class="DigNum (strict)"("DisabledEnum"=w1513) -> ()  [unwired: 2 in, 2 out]
            n287 = property on="Save As Preset" class="Bool"("DisabledEnum"=w1517) -> ()  [unwired: 2 in, 2 out]
            n288 = property on="Line Scan Settings" class="Clust (strict)"("DisabledEnum"=w1517) -> ()  [unwired: 2 in, 2 out]
          }
          event "Line Scanning Presets": Value Change {
            n289 = event-data() -> ("CtlRef"=w1542:refnum<vi>)  [unwired: 1 in]
            n290 = control-ref of="This VI"() -> (w1546:refnum<vi>)
            n291 = property class="Ring (strict)"(reference=w1542) -> ("RingText.Text"=w1540:string)  [unwired: 1 in, 2 out]
            n292 = property class="VI"(reference=w1546) -> ("Path"=w1545:path)  [unwired: 1 in, 2 out]
            n293 = Strip Path(path=w1545) -> (stripped path=w1544:path)  [unwired: 1 out]
            n294 = Concatenate Strings(w1540, ".json" ("string")) -> (w1538:string)
            n295 = Build Path(base path=w1544, name or relative path="4Pi Capture Manager Line Scan Presets") -> (appended path=w1541:path)
            n296 = Build Path(base path=w1541, name or relative path=w1538) -> (appended path=w1537:path)
            n297 = Read from Text File(file (use dialog)=w1537) -> (text=w1536:string, error out=w1534:errorcluster)  [unwired: 3 in, 2 out]
            n298 = Unflatten From JSON(JSON string=w1536, type and defaults=T4 {"Interline Interval"=0.0, "Offset (V)"=0.0, "Amplitude (V)"=0.0, "Samples Per Channel"=0.0, "Delay (ms)"=0.0} ("Line Scan Settings"), error in (no error)=w1534) -> (value=w1533:T4)  [unwired: 4 in, 1 out]
            n299 = property on="Line Scan Settings" class="Clust (strict)"("Val(Sgnl)"=w1533) -> ()  [unwired: 2 in, 2 out]
          }
          event Value Change {
            # "If you try and set the ILI while the camera is in area mode it gives an error"
            n300 = event-data() -> ("NewVal"=w1560:T4)  [unwired: 1 in]
            n301 = Get Notifier Status(notifier=w1565) -> (current notification=w1564:T12)  [unwired: 1 in, 4 out]
            n302 = Unbundle By Name(w1560) -> ("Offset (V)"=w1554:dbl, "Amplitude (V)"=w1558:dbl, "Samples Per Channel"=w1557:dbl, "Delay (ms)"=w1556:dbl, "Interline Interval"=w1550:dbl)
            n303 = Unbundle By Name(w1564) -> ("Line Scan?"=w1549:bool)
            n304 = To Long Integer(number=w1557) -> (32bit integer=w1555:i32)
            n305 = Select(t=w1554, s=w1549, f=0.0) -> (s? t:f=w1552:dbl)
            n306 = Select(t=AO_SCTR_Actions."Update and Run" ("Actions"), s=w1549, f=AO_SCTR_Actions."Stop at Offset" ("Actions")) -> (s? t:f=w1561:T31)
            n307 = call "AO SCTR Messenger.vi"("Notifier Name"=w1559, "Actions"=w1561, "Offset (V)"=w1552, "Amplitude (V)"=w1558, "Samples Per Channel"=w1555, "Start Delay (ms)"=w1556) -> ()  [unwired: 9 in, 1 out]
            n308 = case shown="True" w1549 {
              tunnel: w1551 -> [_ w1570]
              tunnel: w1550 -> [_ w1569]
              frame False {
              }
              frame True {
                n309 = Bundle By Name(cluster=T19 {"Value"=0.0, "Orca Flash Parameters"=4226016} ("sCMOS Parameter"), "Value"=w1569) -> (w1573:T19)
                n310 = call "Orca Flash Messanger.vi"("Notifier Name"=w1570, "Camera Actions"=Orca_Flash_Actions."SETPARAM", "sCMOS Parameter"=w1573) -> ("sCMOS Parameter"=w1574:T19)  [unwired: 8 in, 4 out]
                n311 = Unbundle By Name(w1574) -> ("Value"=w1568:dbl)
                n312 = property on="Interline Interval" class="DigNum (strict)"("Value"=w1568) -> ()  [unwired: 2 in, 2 out]
              }
            }
          }
          event "Save As Preset": Value Change {
            n313 = event-data() -> ()  [unwired: 1 in, 6 out]
            n314 = control-ref of="This VI"() -> (w1587:refnum<vi>)
            n315 = property class="VI"(reference=w1587) -> ("Path"=w1586:path)  [unwired: 1 in, 2 out]
            n316 = Strip Path(path=w1586) -> (stripped path=w1585:path)  [unwired: 1 out]
            n317 = Build Path(base path=w1585, name or relative path="4Pi Capture Manager Line Scan Presets") -> (appended path=w1576:path)
            n318 = call "File Dialog"("start path"=w1576, "prompt"="Save Preset File", "pattern (all files)"="*.json", "pattern label"="JSON") -> ("selected path"=w1581:path, "error out"=w1582:errorcluster)  [unwired: 8 in, 2 out]
            n319 = case shown="Error" w1582 {
              selector: w1582 -> [_ w1605]
              tunnel: w1581 -> [w1604 _]
              tunnel: [w1600 w1605] -> w1575
              frame No Error {
                n320 = local read "Line Scan Settings"() -> (w1603:T4)
                n321 = Flatten To JSON(anything=w1603) -> (JSON string=w1602:string, 11:w1601:errorcluster)  [unwired: 2 in]
                n322 = Write to Text File(file (use dialog)=w1604, text=w1602, error in=w1601) -> (error out=w1600:errorcluster)  [unwired: 1 in, 2 out]
              }
              frame Error {
              }
            }
            n323 = List Folder(path=w1576, pattern="*.json", error in=w1575) -> (filenames=w1579:string[], error out=w1578:errorcluster)  [unwired: 1 in, 2 out]
            n324 = case shown="No Error" w1578 {
              tunnel: w1579 -> [w1594 _]
              tunnel: w1576 -> [w1593 _]
              tunnel: [w1592 string[] []] -> w1577
              frame No Error {
                n325 = for {
                  tunnel: w1594 -> [w1597] mode=indexing
                  tunnel: w1593 -> [w1598]
                  tunnel: [w1595] -> w1592 mode=indexing
                  n326 = Build Path(base path=w1598, name or relative path=w1597) -> (appended path=w1596:path)
                  n327 = call <vilib>:"Get File Extension.vi"("file"=w1596) -> ("filename without extension"=w1595:string)  [unwired: 6 in, 4 out]
                }
              }
              frame Error {
              }
            }
            n328 = property on="Line Scanning Presets" class="Ring (strict)"("Strings []"=w1577) -> ()  [unwired: 2 in, 2 out]
          }
          event "Quit": Value Change {
            n329 = event-data() -> ("NewVal"=w1620:bool)  [unwired: 1 in]
            n330 = Get Notifier Status(notifier=w1619) -> (notifier out=w1618:refnum<notifier>, current notification=w1617:T12)  [unwired: 1 in, 3 out]
            n331 = Bundle By Name(cluster=w1617, "Running?"=FALSE ("Abort"), "Actions"=4Pi_Capture_Actions."Quit") -> (w1611:T12)
            n332 = Send Notification(notification=w1611, notifier=w1618) -> (notifier out=w1615:refnum<notifier>)  [unwired: 1 in, 1 out]
            n333 = Wait on Notification(notifier=w1615, ignore previous (F)=TRUE, timeout in ms (-1)=500) -> (notifier out=w1612:refnum<notifier>)  [unwired: 1 in, 3 out]
            n334 = Send Notification(notification=w1611, notifier=w1612) -> (notifier out=w1609:refnum<notifier>)  [unwired: 1 in, 1 out]
            n335 = Release Notifier(notifier=w1609, force destroy? (F)=TRUE) -> ()  [unwired: 1 in, 3 out]
            n336 = for {
              tunnel: w1607 -> [w1621] mode=indexing
              n337 = call "IMAQ Dispose"("Image"=w1621) -> ()  [unwired: 5 in, 1 out]
            }
          }
        }
      }
      n338 = while {
        tunnel: w232 -> [w275]
        tunnel: w201 -> [w269]
        tunnel: w231 -> [w267]
        tunnel: w230 -> [w266]
        tunnel: w229 -> [w265]
        tunnel: [FALSE] -> w228
        tunnel: w222 -> [w263]
        tunnel: w195 -> [w258]
        tunnel: w194 -> [w257]
        tunnel: w186 -> [w256]
        tunnel: [w256] -> w185
        tunnel: w173 -> [w253]
        stop <- w271 stop-if-true
        w254 = u16 0 ("Current Mode")
        w261 = u16 0 ("Current Step")
        n339 = Wait on Notification(notifier=w275, ignore previous (F)=TRUE) -> (notifier out=w270:refnum<notifier>, notification=w273:T12)  [unwired: 2 in, 2 out]
        n340 = Unbundle By Name(w273) -> ("Actions"=w268:T13)
        n341 = Bundle By Name(cluster=T24 {"Current Step"=0, "Current Cycle"=0, "Current Laser"=0, "# of Lasers"=0, "# of Cycles"=0, "# of Steps"=0, "Switch Laser At"=enum."All Cycles", "Current Mirror Mode"=0, "# of Mirror Mode"=0, "Current Amp step"=0, "# of Amp steps"=0} ("Cluster"), "Current Step"=w261, "Current Cycle"=w261, "Current Laser"=w261, "# of Lasers"=u16 1, "Switch Laser At"="Switch Laser At", "Current Mirror Mode"=w254, "Current Amp step"=w254) -> (w260:T24)
        n342 = Equal?(x=w268, y=4Pi_Capture_Actions."Quit") -> (x = y?=w271:bool)
        n343 = while {
          shift-right: [w291] -> _
          shift-left: w268 -> [w292]
          tunnel: w270 -> [w283]
          tunnel: w269 -> [w288]
          tunnel: w268 -> [w287]
          tunnel: w267 -> [w286]
          tunnel: w266 -> [w285]
          tunnel: w265 -> [w284]
          tunnel: w263 -> [w282]
          shift-right: [w280] -> _
          shift-left: w260 -> [w281]
          tunnel: w258 -> [w279]
          tunnel: w257 -> [w278]
          tunnel: w256 -> [w277]
          tunnel: w253 -> [w276]
          stop <- w289 stop-if-true
          n344 = case shown="\"Write Metadata\"" w292 {
            selector: w292 -> [_ _ _ w391 w420 _ _ _ _ _ _ _ _ _ _ _ _ _ _]
            tunnel: [4Pi_Capture_Actions."Quit" ("y") 4Pi_Capture_Actions."Open Shutters" ("y") 4Pi_Capture_Actions."Close Shutters" ("y") w382 w414 4Pi_Capture_Actions."Start Acquisition" ("y") w490 4Pi_Capture_Actions."Write Metadata" ("y") w601 w656 w690 w735 w829 w861 w889 w966 w1019 w1138 4Pi_Capture_Actions."Quit" ("y")] -> w291
            tunnel: [w294 w306 w344 w393 w418 w449 w492 w569 w631 w665 w699 w765 w855 w860 w904 w985 w1036 w1160 TRUE] -> w289
            tunnel: FALSE -> [w294 w306 w344 w393 w418 w449 w492 w569 w631 w665 w699 w765 w855 w860 w904 w985 w1036 w1160 _]
            tunnel: w288 -> [_ w299 w338 _ w410 w434 w491 _ _ _ w689 w757 _ _ _ _ _ _ _]
            tunnel: w287 -> [_ _ w337 _ _ w442 w488 w566 w623 _ _ _ _ _ _ _ _ _ _]
            tunnel: w286 -> [_ _ _ _ w417 _ _ _ _ _ _ _ _ _ _ _ _ _ _]
            tunnel: w285 -> [_ _ _ w392 _ _ _ _ _ _ _ _ _ _ _ _ _ _ _]
            tunnel: w284 -> [_ _ _ w387 _ _ _ _ _ _ _ _ _ _ _ _ _ _ _]
            tunnel: w283 -> [_ _ w335 _ _ w447 w489 w568 w624 _ w691 w758 w835 _ w903 w984 w1035 _ _]
            tunnel: w282 -> [_ _ w332 _ _ _ w487 _ _ _ _ _ _ _ w901 w977 _ _ _]
            tunnel: w281 -> [w293 w305 w316 w380 w412 w437 w486 w567 w598 w664 w684 w733 w833 w868 w894 w971 w1026 w1159 w1182]
            tunnel: [w293 w305 w316 w380 w412 w437 w483 w567 w598 w664 w684 w732 w854 w867 w894 w971 w1026 w1159 w1182] -> w280
            tunnel: w279 -> [_ _ _ _ _ w430 _ _ _ _ _ _ _ _ _ _ _ _ _]
            tunnel: w278 -> [_ _ _ _ _ w429 _ _ _ _ _ _ _ _ _ _ _ _ _]
            tunnel: w277 -> [_ w304 w311 _ _ _ w485 _ _ _ w679 w750 _ _ _ w975 _ _ _]
            tunnel: w276 -> [_ _ _ _ _ _ w484 _ _ _ _ _ _ _ _ _ _ _ _]
            frame "Idle", Default {
            }
            frame "Live Preview", "Capture" {
              w296 = FALSE ("Camera Running?")
              n345 = call "Orca Flash Messanger.vi"("Notifier Name"=w299, "Camera Actions"=Orca_Flash_Actions."STATUS") -> ("Image Ref"=w298:T8)  [unwired: 9 in, 4 out]
              n346 = Get Notifier Status(notifier=w304) -> (notifier out=w302:refnum<notifier>, current notification=w303:T9)  [unwired: 1 in, 3 out]
              n347 = Bundle By Name(cluster=w303, "Image Ref"=w298, "Cycle Number"=u16 0, "Camera Running?"=w296, "Capture?"=w296) -> (w301:T9)
              n348 = Send Notification(notification=w301, notifier=w302) -> ()  [unwired: 1 in, 2 out]
            }
            frame "Abort" {
              w315 = FALSE ("Capture?")
              w331 = u16 1 ("Current Cycle")
              w339 = FALSE ("Live Preview")
              n349 = call "Orca Flash Messanger.vi"("Notifier Name"=w338, "Camera Actions"=Orca_Flash_Actions."IDLE") -> ()  [unwired: 9 in, 5 out]
              n350 = local write "Live Preview"(w339) -> ()
              n351 = local write "Capture"(w339) -> ()
              n352 = Equal?(x=4Pi_Capture_Actions."Capture", y=w337) -> (x = y?=w317:bool)
              n353 = Get Notifier Status(notifier=w335) -> (notifier out=w342:refnum<notifier>, current notification=w341:T12)  [unwired: 1 in, 3 out]
              n354 = Bundle By Name(cluster=w341, "Running?"=FALSE) -> (w334:T12)
              n355 = local write "Current Cycle"(w331) -> ()
              n356 = local write "Current Step"(w331) -> ()
              n357 = Get Notifier Status(notifier=w311) -> (notifier out=w314:refnum<notifier>, current notification=w313:T9)  [unwired: 1 in, 3 out]
              n358 = Bundle By Name(cluster=w313, "Camera Running?"=w315, "Capture?"=w315) -> (w312:T9)
              n359 = Send Notification(notification=w334, notifier=w342) -> ()  [unwired: 1 in, 2 out]
              n360 = Unbundle By Name(w334) -> ("Init Mirror Modes"=w308:T14, "Metadata File Ref"=w309:refnum<file>[], "Init Z Position (µm)"=w333:dbl)
              n361 = Obtain Notifier(name (unnamed)="WFDC External Sync", notification data type=T26 {"Cycle Sync"=enum."Pause Requested", "Z Offset"=0.0, "WFDC Status"=enum."Idle"} ("WFDC External Sync"), create if not found? (T)=FALSE) -> (notifier out=w327:refnum<notifier>, error out=w321:errorcluster)  [unwired: 1 in, 1 out]
              n362 = Send Notification(notification=w312, notifier=w314) -> ()  [unwired: 1 in, 2 out]
              n363 = Get Notifier Status(notifier=w327, error in (no error)=w321) -> (notifier out=w319:refnum<notifier>, current notification=w318:T26, error out=w322:errorcluster)  [unwired: 2 out]
              n364 = Unbundle By Name(w318) -> ("WFDC Status"=w326:T25)
              n365 = Unbundle By Name(w322) -> ("status"=w323:bool)
              n366 = Not A Number/Path/Refnum?(number/path/refnum=w309) -> (NaN/Path/Refnum?=w310:bool[])
              n367 = for {
                tunnel: w310 -> [w347] mode=indexing
                tunnel: w309 -> [w346] mode=indexing
                n368 = case shown="False" w347 {
                  tunnel: w346 -> [w348 _]
                  frame False {
                    n369 = Close File(refnum=w348) -> ()  [unwired: 1 in, 2 out]
                  }
                  frame True {
                  }
                }
              }
              n370 = Not Equal?(x=WFDC_Status."DC Active", y=w326) -> (x != y?=w324:bool)
              n371 = Or(x=w324, y=w323) -> (x .or. y?=w320:bool)
              n372 = case shown="True" w317 {
                tunnel: w333 -> [_ w358]
                tunnel: w332 -> [_ w357]
                tunnel: w320 -> [_ w356]
                tunnel: w319 -> [_ w355]
                tunnel: w318 -> [_ w354]
                tunnel: w308 -> [_ w349]
                frame False {
                }
                frame True {
                  w350 = 4Pi_Dual_DM_-_Standard_Action."Read" ("Action")
                  n373 = case shown="True" w356 {
                    tunnel: w358 -> [_ w379]
                    tunnel: w357 -> [_ w378]
                    tunnel: w355 -> [w372 _]
                    tunnel: w354 -> [w371 _]
                    frame False {
                      n374 = Bundle By Name(cluster=w371, "Z Offset"=0.0) -> (w373:T26)
                      n375 = Send Notification(notification=w373, notifier=w372) -> (notifier out=w368:refnum<notifier>)  [unwired: 1 in, 1 out]
                      n376 = Release Notifier(notifier=w368, force destroy? (F)=FALSE) -> ()  [unwired: 1 in, 3 out]
                    }
                    frame True {
                      n377 = Build Array(w379) -> (w374:dbl[])
                      n378 = call "Stages Messenger.vi"("Stage Notifier Name"=w378, "Actions"=Stage_Actions."MOVE", "Setpoint"=w374, "Axis"=bool[] [TRUE], "Exit While Busy?"=FALSE) -> ()  [unwired: 6 in, 5 out]
                    }
                  }
                  n379 = call "4Pi Dual DM - Mirror Mode DUAL AE.vi"("Action"=w350) -> ("Mirror Modes Out"=w352:T36)  [unwired: 14 in]
                  n380 = call "4Pi Dual DM - Active Mirror AE.vi"("Action"=w350) -> ("Active Mirror"=w351:i32)  [unwired: 14 in]
                  n381 = Replace Array Subset(array=w352, new element=w349, index (col)=w351) -> (w353:T36)  [unwired: 1 in]
                  n382 = flat-sequence {
                    tunnel: w353 -> [w359]
                    frame #0 {
                      n383 = call "4Pi Dual DM - Mirror Mode DUAL AE.vi"("Action"=4Pi_Dual_DM_-_Standard_Action."Write", "Mirror Modes In"=w359) -> ()  [unwired: 13 in, 1 out]
                    }
                    frame #1 {
                      w365 = "Mirror Control Que" ("name (unnamed)")
                      n384 = Obtain Queue(max queue size (-1, unlimited)=10, name (unnamed)=w365, element data type=w365, create if not found? (T)=FALSE) -> (queue out=w361:refnum<queue>, error out=w362:errorcluster)  [unwired: 1 in, 1 out]
                      n385 = case shown="No Error" w362 {
                        tunnel: w361 -> [w366 _]
                        frame No Error {
                          n386 = Enqueue Element(queue=w366, element="Mirror Modes" ("name (unnamed)")) -> ()  [unwired: 2 in, 3 out]
                        }
                        frame Error {
                        }
                      }
                    }
                  }
                }
              }
            }
            frame "Open Shutters", "Close Shutters" {
              n387 = Equal?(x=w391, y=4Pi_Capture_Actions."Open Shutters") -> (x = y?=w385:bool)
              n388 = Select(t=Shutter_Actions."Open" ("Action"), s=w385, f=Shutter_Actions."Close") -> (s? t:f=w386:T29)
              n389 = case shown="False" "Auto Shutter" {
                tunnel: w392 -> [_ w400]
                tunnel: w387 -> [_ w395]
                tunnel: w386 -> [_ w394]
                frame False {
                }
                frame True {
                  n390 = flat-sequence {
                    tunnel: w394 -> [w403]
                    tunnel: w400 -> [w404]
                    tunnel: [w404] -> w397
                    tunnel: [w403] -> w396
                    tunnel: w395 -> [w402]
                    tunnel: w394 -> [w401]
                    tunnel: [w407] -> w399
                    tunnel: [w406] -> w398
                    tunnel: w397 -> [w407]
                    tunnel: w396 -> [w406]
                    tunnel: w399 -> [w409]
                    tunnel: w398 -> [w408]
                    frame #0 {
                      n391 = call "Shutter Messenger.vi"("Notifier Name"=w402, "Action"=w401) -> ()  [unwired: 12 in, 2 out]
                    }
                    frame #1 {
                      n392 = Wait (ms)(milliseconds to wait=u32 100) -> ()  [unwired: 1 out]
                    }
                    frame #2 {
                      n393 = call "Shutter Messenger.vi"("Notifier Name"=w409, "Action"=w408) -> ()  [unwired: 12 in, 2 out]
                    }
                  }
                }
              }
              n394 = Select(t=4Pi_Capture_Actions."Laser On" ("y"), s=w385, f=4Pi_Capture_Actions."Laser Off") -> (s? t:f=w382:T13)
            }
            frame "Laser On", "Laser Off" {
              n395 = Equal?(x=w420, y=4Pi_Capture_Actions."Laser On") -> (x = y?=w411:bool)
              n396 = call "AOTF Messenger.vi"("AOTF Notifier Name"=w417, "AOTF Action"=AOTF_Actions."Blank", "Beam Blank"=w411) -> ()  [unwired: 7 in, 6 out]
              n397 = disable-structure shown="Disabled" {
                disable-tunnel: w411 -> [w422 _]
                disable-tunnel: w410 -> [w421 _]
                frame Disabled {
                  n398 = case shown="True" w422 {
                    tunnel: w421 -> [w424 w427]
                    frame False {
                      n399 = call "Orca Flash Messanger.vi"("Notifier Name"=w424, "Camera Actions"=Orca_Flash_Actions."SETPARAM", "sCMOS Parameter"=T19 {"Value"=2.0, "Orca Flash Parameters"=1853168}) -> ()  [unwired: 8 in, 5 out]
                    }
                    frame True {
                      n400 = call "Orca Flash Messanger.vi"("Notifier Name"=w427, "Camera Actions"=Orca_Flash_Actions."SETPARAM", "sCMOS Parameter"=T19 {"Value"=5.0, "Orca Flash Parameters"=1853168}) -> ()  [unwired: 8 in, 5 out]
                    }
                  }
                }
                frame Enabled {
                }
              }
              n401 = Select(t=4Pi_Capture_Actions."Set Exposure Time" ("y"), s=w411, f=4Pi_Capture_Actions."Quit" ("y")) -> (s? t:f=w414:T13)
            }
            frame "Set Exposure Time" {
              # "Frame Rate (Hz)"
              n402 = Get Notifier Status(notifier=w447) -> (current notification=w443:T12)  [unwired: 1 in, 4 out]
              n403 = Unbundle By Name(w443) -> ("Line Scan?"=w432:bool, "Line Scan Mode"=w431:T3, "Capture Exposure (s)"=w438:dbl, "Preview Exposure (s)"=w439:dbl)
              n404 = Equal?(x=w442, y=4Pi_Capture_Actions."Capture") -> (x = y?=w440:bool)
              n405 = Select(t=w438, s=w440, f=w439) -> (s? t:f=w436:dbl)
              n406 = case shown="True" w432 {
                tunnel: w436 -> [w451 w459]
                tunnel: [w451 w456] -> w435
                tunnel: w434 -> [w450 w458]
                tunnel: [w450 w455] -> w433
                tunnel: w431 -> [_ w454]
                tunnel: w430 -> [_ w453]
                tunnel: w429 -> [_ w452]
                frame False {
                  # "Exposure Time (s)"
                }
                frame True {
                  n407 = To Double Precision Float(number="Number of Lines") -> (double precision float=w457:dbl)
                  n408 = case shown="Default" w454 {
                    tunnel: w459 -> [_ w482]
                    tunnel: w458 -> [w465 w481]
                    tunnel: w457 -> [w463 w480]
                    tunnel: [w461 w479] -> w456
                    tunnel: [w464 w478] -> w455
                    tunnel: w453 -> [_ w471]
                    tunnel: w452 -> [_ w470]
                    frame Default {
                      n409 = call "Orca Flash Messanger.vi"("Notifier Name"=w465, "Camera Actions"=Orca_Flash_Actions."GETPARAM", "sCMOS Parameter"=T19 {"Value"=0.0, "Orca Flash Parameters"=4226016}) -> ("Notifier Name Dup"=w464:string, "sCMOS Parameter"=w468:T19)  [unwired: 8 in, 3 out]
                      n410 = Unbundle By Name(w468) -> ("Value"=w462:dbl)
                      n411 = Multiply(x=w462, y=w463) -> (x*y=w461:dbl)
                    }
                    frame "Automatic" {
                      n412 = call "4Pi Capture Set Interline Interval.vi"("Camera Notifier Name"=w481, "Frame Rate (Hz)"=w482) -> ("Camera Notifier Name (Dup)"=w478:string, "Interline Interval (s)"=w477:dbl)  [unwired: 12 in]
                      n413 = Multiply(x=w477, y=w480) -> (x*y=w479:dbl)
                      n414 = call "4Pi Capture Set Auto Waveform.vi"("Interline Interval"=w477, "Waveform Parameters"=w470) -> ("Offset (V)"=w475:dbl, "Amplitude (V)"=w474:dbl, "Samples per Channel"=w473:i32, "Delay (ms)"=w472:dbl, "Line Scan Settings"=w469:T4)  [unwired: 9 in]
                      n415 = local write "Line Scan Settings"(w469) -> ()
                      n416 = call "AO SCTR Messenger.vi"("Notifier Name"=w471, "Actions"=AO_SCTR_Actions."Update and Run", "Offset (V)"=w475, "Amplitude (V)"=w474, "Samples Per Channel"=w473, "Start Delay (ms)"=w472) -> ()  [unwired: 9 in, 1 out]
                    }
                  }
                }
              }
              n417 = Bundle By Name(cluster=T19 {"Value"=0.0, "Orca Flash Parameters"=2049184} ("sCMOS Parameter"), "Value"=w435) -> (w446:T19)
              n418 = call "Orca Flash Messanger.vi"("Notifier Name"=w433, "Camera Actions"=Orca_Flash_Actions."SETPARAM", "sCMOS Parameter"=w446) -> ()  [unwired: 8 in, 5 out]
            }
            frame "Start Acquisition" {
              n419 = case shown="\"Capture\"" w488 {
                tunnel: w491 -> [_ w495 _]
                tunnel: [4Pi_Capture_Actions."Quit" ("y") 4Pi_Capture_Actions."Quit" ("y") 4Pi_Capture_Actions."Update SubFolder" ("y")] -> w490
                tunnel: w489 -> [_ _ w540]
                tunnel: w487 -> [_ _ w532]
                tunnel: w486 -> [w493 w496 w528]
                tunnel: [w493 w496 w527] -> w483
                tunnel: w485 -> [_ _ w523]
                tunnel: w484 -> [_ _ w501]
                frame Default {
                }
                frame "Live Preview" {
                  n420 = call "Orca Flash Messanger.vi"("Notifier Name"=w495, "Camera Actions"=Orca_Flash_Actions."PREVIEW") -> ()  [unwired: 9 in, 5 out]
                }
                frame "Capture" {
                  w504 = 4Pi_Dual_DM_-_Standard_Action."Read" ("Action")
                  w526 = sgl 0.0 ("Cycle")
                  n421 = Get Notifier Status(notifier=w523) -> (notifier out=w524:refnum<notifier>, current notification=w522:T9)  [unwired: 1 in, 3 out]
                  n422 = Bundle By Name(cluster=w522, "Capture?"=TRUE) -> (w521:T9)
                  n423 = call "Stages Messenger.vi"("Stage Notifier Name"=w532, "Actions"=Stage_Actions."Get Position") -> ("Positions"=w535:dbl[])  [unwired: 9 in, 4 out]
                  n424 = Send Notification(notification=w521, notifier=w524) -> ()  [unwired: 1 in, 2 out]
                  n425 = Index Array(array=w535, index=0) -> (element=w533:dbl)
                  n426 = call "4Pi Dual DM - Mirror Mode DUAL AE.vi"("Action"=w504) -> ("Mirror Modes Out"=w505:T36)  [unwired: 14 in]
                  n427 = call "4Pi Dual DM - Active Mirror AE.vi"("Action"=w504) -> ("Active Mirror"=w506:i32)  [unwired: 14 in]
                  n428 = call "Stages Messenger.vi"("Stage Notifier Name"=w501, "Actions"=Stage_Actions."SERVO ON/OFF", "Servo On?"=FALSE, "Exit While Busy?"=FALSE) -> ()  [unwired: 7 in, 5 out]
                  n429 = Index Array(array=w505, index (col)=w506) -> (element=w503:cluster{"Mode":string, "Amplitude":dbl}[])  [unwired: 1 in]
                  n430 = Get Notifier Status(notifier=w540) -> (notifier out=w537:refnum<notifier>, current notification=w538:T12)  [unwired: 1 in, 3 out]
                  n431 = Bundle By Name(cluster=w538, "Init Mirror Modes"=w503, "Init Z Position (µm)"=w533) -> (w529:T12)
                  n432 = Unbundle By Name(w529) -> ("No. Amp steps"=w508:u16, "No. Mirror Mode"=w507:u16, "Cycles"=w530:u16, "No. of Z Steps"=w531:u16)
                  n433 = Send Notification(notification=w529, notifier=w537) -> ()  [unwired: 1 in, 2 out]
                  n434 = local write "Z Step"(w526) -> ()
                  n435 = local write "Cycle"(w526) -> ()
                  n436 = local write "Frame"(u32 0 ("Frame")) -> ()
                  n437 = Bundle By Name(cluster=w528, "# of Amp steps"=w508, "# of Mirror Mode"=w507, "# of Cycles"=w530, "# of Steps"=w531) -> (w527:T24)
                  n438 = Obtain Notifier(name (unnamed)="WFDC External Sync", notification data type=T26 {"Cycle Sync"=enum."Pause Requested", "Z Offset"=0.0, "WFDC Status"=enum."Idle"} ("WFDC External Sync"), create if not found? (T)=FALSE) -> (notifier out=w510:refnum<notifier>, error out=w509:errorcluster)  [unwired: 1 in, 1 out]
                  n439 = Get Notifier Status(notifier=w510, error in (no error)=w509) -> (notifier out=w515:refnum<notifier>, current notification=w516:T26, error out=w517:errorcluster)  [unwired: 2 out]
                  n440 = Unbundle By Name(w516) -> ("WFDC Status"=w514:T25)
                  n441 = case shown="\"Error\"" w514 {
                    tunnel: w515 -> [w543 w548]
                    tunnel: w516 -> [_ w547]
                    tunnel: w517 -> [w542 w545]
                    tunnel: [w543 w546] -> w519
                    tunnel: [w542 w544] -> w518
                    frame Default {
                    }
                    frame "Error" {
                      n442 = Two Button Dialog(message="Reset Wide Field Drift Correction error?", 1:"No" ("F button name (\"Cancel\")"), 2:"Yes" ("T button name (\"OK\")")) -> (T button?=w552:bool)
                      n443 = case shown="True" w552 {
                        tunnel: w548 -> [w554 w559]
                        tunnel: w547 -> [_ w561]
                        tunnel: [w554 w557] -> w546
                        tunnel: w545 -> [w553 w556]
                        tunnel: [w553 w555] -> w544
                        frame False {
                        }
                        frame True {
                          n444 = Bundle By Name(cluster=w561, "WFDC Status"=WFDC_Status."Idle") -> (w558:T26)
                          n445 = Send Notification(notification=w558, notifier=w559, error in (no error)=w556) -> (notifier out=w557:refnum<notifier>, error out=w555:errorcluster)
                        }
                      }
                    }
                  }
                  n446 = case shown="Error" w518 {
                    tunnel: w519 -> [w541 _]
                    frame No Error {
                      n447 = Release Notifier(notifier=w541) -> ()  [unwired: 2 in, 3 out]
                    }
                    frame Error {
                    }
                  }
                }
              }
            }
            frame "Update SubFolder" {
              n448 = Equal?(x=w566, y=4Pi_Capture_Actions."Capture") -> (x = y?=w564:bool)
              n449 = And(x=w564, y="Auto Update Subfolder") -> (x .and. y?=w562:bool)
              n450 = case shown="True" w562 {
                tunnel: w568 -> [w575 w591]
                frame False {
                  n451 = Get Notifier Status(notifier=w575) -> (notifier out=w574:refnum<notifier>, current notification=w572:T12)  [unwired: 1 in, 3 out]
                  n452 = Unbundle By Name(w572) -> ("Base Path"=w571:path)
                  n453 = Bundle By Name(cluster=w572, "Save Path"=w571) -> (w573:T12)
                  n454 = Send Notification(notification=w573, notifier=w574) -> ()  [unwired: 1 in, 2 out]
                }
                frame True {
                  n455 = Get Notifier Status(notifier=w591) -> (notifier out=w579:refnum<notifier>, current notification=w578:T12)  [unwired: 1 in, 3 out]
                  n456 = feedback #1(u32 0) -> (w581:u32)
                  n457 = Unbundle By Name(w578) -> ("Base Path"=w590:path)
                  n458 = Increment(x=w581) -> (x+1=w580:u32)
                  n459 = feedback-in #1(w580) -> ()
                  n460 = Format Into String(format string="%03d", w580) -> (resulting string=w582:string)  [unwired: 2 in, 1 out]
                  n461 = Strip Path(path=w590) -> (stripped path=w589:path, name=w587:string)
                  n462 = Concatenate Strings("Subfolder Name", w582) -> (w585:string)
                  n463 = Build Path(base path=w589, name or relative path=w585) -> (appended path=w588:path)
                  n464 = Build Path(base path=w588, name or relative path=w587) -> (appended path=w577:path)
                  n465 = Bundle By Name(cluster=w578, "Save Path"=w577) -> (w576:T12)
                  n466 = Send Notification(notification=w576, notifier=w579) -> ()  [unwired: 1 in, 2 out]
                }
              }
            }
            frame "Write Metadata" {
              w603 = T5 0 items=["Idle", "Orthogonal", "Random"] ("y")
              w619 = T5 2 items=["Idle", "Orthogonal", "Random"] ("y")
              n467 = Get Notifier Status(notifier=w624) -> (notifier out=w622:refnum<notifier>, current notification=w606:T12)  [unwired: 1 in, 3 out]
              n468 = Not Equal?(x=4Pi_Capture_Actions."Capture", y=w623) -> (x != y?=w610:bool)
              n469 = Unbundle By Name(w606) -> ("Init Z Position (µm)"=w621:dbl, "Save Path"=w595:path, "Z Step Size (µm)"=w628:dbl, "No. of Z Steps"=w627:u16, "DM scan mode"=w620:T5)
              n470 = Equal?(x=w620, y=w619) -> (x = y?=w609:bool)
              n471 = Not(x=w609) -> (.not. x?=w608:bool)
              n472 = Less?(x=w627, y=u16 2) -> (x < y?=w625:bool)
              n473 = Equal To 0?(x=w628) -> (x = 0?=w626:bool)
              n474 = Compound Arithmetic op=OR(w626, w625, w610) -> (w611:bool)
              n475 = Compound Arithmetic op=OR(w608, w610) -> (w607:bool)
              n476 = Strip Path(path=w595) -> (stripped path=w615:path, name=w593:string)
              n477 = call <vilib>:"Check if File or Folder Exists.vi"("path"=w615) -> ("file or folder exists?"=w617:bool, "dup path"=w616:path)  [unwired: 8 in, 1 out]
              n478 = case shown="False" w617 {
                tunnel: [w653 w655] -> w594
                tunnel: w616 -> [w654 w655]
                frame False {
                  n479 = Create Folder(path (use dialog)=w654) -> (created path=w653:path)  [unwired: 2 in, 2 out]
                }
                frame True {
                }
              }
              n480 = case shown="False" w607 {
                tunnel: [w633 refnum<k0> refnum] -> w613
                tunnel: w594 -> [w632 _]
                frame False {
                  n481 = Build Path(base path=w632, name or relative path="DM Amplitude.txt") -> (appended path=w635:path)
                  n482 = Open/Create/Replace File(file path (use dialog)=w635, operation (0:open)=T32."replace or create") -> (refnum out=w633:refnum<file>)  [unwired: 4 in, 2 out]
                }
                frame True {
                }
              }
              n483 = case shown="False" w611 {
                tunnel: w621 -> [w649 _]
                tunnel: w594 -> [w639 _]
                tunnel: [w638 refnum<k0> refnum] -> w614
                frame False {
                  n484 = Build Path(base path=w639, name or relative path="Z Positions.txt") -> (appended path=w647:path)
                  n485 = Open/Create/Replace File(file path (use dialog)=w647, operation (0:open)=T32."replace or create") -> (refnum out=w644:refnum<file>, error out=w642:errorcluster)  [unwired: 4 in, 1 out]
                  n486 = Format Value(format string="%.4f\\n", value (0)=w649) -> (output string=w643:string)  [unwired: 1 in]
                  n487 = Write to Text File(file (use dialog)=w644, text=w643, error in=w642) -> (refnum out=w640:refnum<file>, error out=w641:errorcluster)  [unwired: 1 in, 1 out]
                  n488 = case shown="No Error" w641 {
                    tunnel: w640 -> [w650 _]
                    tunnel: [w650 refnum<k0> refnum] -> w638
                    frame No Error {
                    }
                    frame Error {
                    }
                  }
                }
                frame True {
                }
              }
              n489 = Build Path(base path=w594, name or relative path=w593) -> (appended path=w592:path)
              n490 = call "4Pi Capture Write Meta Data.vi"("data path"=w592) -> ()  [unwired: 11 in]
              n491 = Build Array(w614, w613) -> (w612:refnum<file>[])
              n492 = Bundle By Name(cluster=w606, "Metadata File Ref"=w612) -> (w618:T12)
              n493 = local read "Soft trigger"() -> (w599:bool)
              n494 = local read "DM scan mode"() -> (w602:T5)
              n495 = Send Notification(notification=w618, notifier=w622) -> ()  [unwired: 1 in, 2 out]
              n496 = Select(t=4Pi_Capture_Actions."Setup", s=w599, f=4Pi_Capture_Actions."Write DM") -> (s? t:f=w596:T13)
              n497 = Equal?(x=w602, y=w603) -> (x = y?=w605:bool)
              n498 = Select(t=4Pi_Capture_Actions."Setup" ("y"), s=w605, f=w596) -> (s? t:f=w601:T13)
            }
            frame "Setup" {
              w662 = T5 0 items=["Idle", "Orthogonal", "Random"] ("y")
              # "Change lasers here"
              n499 = local read "DM scan mode"() -> (w663:T5)
              n500 = Not Equal?(x=w663, y=w662) -> (x != y?=w660:bool)
              n501 = And(x="Soft trigger", y=w660) -> (x .and. y?=w659:bool)
              n502 = Select(t=4Pi_Capture_Actions."Camera Soft Trigger" ("y"), s=w659, f=4Pi_Capture_Actions."Camera") -> (s? t:f=w656:T13)
            }
            frame "Camera" {
              w671 = T5 1 items=["Idle", "Orthogonal", "Random"] ("y")
              n503 = Get Notifier Status(notifier=w691) -> (notifier out=w698:refnum<notifier>, current notification=w686:T12)  [unwired: 1 in, 3 out]
              n504 = Unbundle By Name(w686) -> ("Save Path"=w694:path, "Frames"=w687:u32)
              n505 = local read "DM scan mode"() -> (w672:T5)
              n506 = Unbundle By Name(w684) -> ("Current Cycle"=w670:u16, "Current Step"=w669:u16, "Current Mirror Mode"=w668:u16, "Current Amp step"=w667:u16)
              n507 = Equal?(x=w672, y=w671) -> (x = y?=w666:bool)
              n508 = property on="Current Laser" class="Ring (strict)"() -> ("RingText.Text"=w685:string)  [unwired: 2 in, 2 out]
              n509 = call "4Pi Capture File Name Increment.vi"("Path In"=w694, "Laser Line"=w685, "Cycle"=w670, "Step"=w669, "Mirror Mode"=w668, "Amp step"=w667, "add DM"=w666) -> ("Path Out"=w695:path)  [unwired: 8 in]
              n510 = Get Notifier Status(notifier=w679) -> (notifier out=w683:refnum<notifier>, current notification=w682:T9)  [unwired: 1 in, 3 out]
              n511 = Bundle By Name(cluster=w682, "Camera Running?"=TRUE) -> (w680:T9)
              n512 = call "Orca Flash Messanger.vi"("Notifier Name"=w689, "Camera Actions"=Orca_Flash_Actions."Record Settings", "Path"=w695, "# of frames"=w687) -> ("Notifier Name Dup"=w697:string)  [unwired: 7 in, 4 out]
              n513 = call "Orca Flash Messanger.vi"("Notifier Name"=w697, "Camera Actions"=Orca_Flash_Actions."RECORD") -> ("Notifier Name Dup"=w692:string, "Image Ref"=w688:T8)  [unwired: 9 in, 3 out]
              n514 = Send Notification(notification=w680, notifier=w683) -> (notifier out=w678:refnum<notifier>)  [unwired: 1 in, 1 out]
              n515 = while {
                tunnel: w692 -> [w724]
                tunnel: [w721] -> w690
                tunnel: w698 -> [w711]
                tunnel: w688 -> [w710]
                tunnel: [w709] -> w674
                tunnel: w678 -> [w709]
                stop <- w717 stop-if-true
                n516 = Get Notifier Status(notifier=w711) -> (current notification=w723:T12)  [unwired: 1 in, 4 out]
                n517 = Unbundle By Name(w723) -> ("Running?"=w716:bool)
                n518 = Wait (ms)(milliseconds to wait=u32 10) -> ()  [unwired: 1 out]
                n519 = call "IMAQ Read Custom Data"("Key"="Image Data", "Image"=w710) -> ("Custom Data Out"=w707:string)  [unwired: 7 in, 2 out]
                n520 = Not(x=w716) -> (.not. x?=w720:bool)
                n521 = Unflatten From JSON(JSON string=w707, type and defaults=T33 {"Frame"=0, "Sensor Height"=0, "Sensor Width"=0, "ROI Height"=0, "ROI Width"=0, "ROI Enable?"=FALSE, "Bit per Pixel"=0} ("Camera IMAQ Key Info")) -> (value=w705:T33)  [unwired: 5 in, 1 out]
                n522 = Unbundle By Name(w705) -> ("Frame"=→"Frame" →"Current Frame":u32)
                n523 = Select(t=Orca_Flash_Actions."STATUS" ("Camera Actions"), s=w716, f=Orca_Flash_Actions."IDLE") -> (s? t:f=w712:T23)
                n524 = call "Orca Flash Messanger.vi"("Notifier Name"=w724, "Camera Actions"=w712) -> ("Running?"=w719:bool)  [unwired: 9 in, 4 out]
                n525 = Not(x=w719) -> (.not. x?=w718:bool)
                n526 = Or(x=w720, y=w718) -> (x .or. y?=w717:bool)
                n527 = Select(t=4Pi_Capture_Actions."Swtich1", s="DM first", f=4Pi_Capture_Actions."Switch" ("y")) -> (s? t:f=w700:T13)
                n528 = Select(t=w700, s=w716, f=4Pi_Capture_Actions."Abort") -> (s? t:f=w721:T13)
              }
              n529 = Get Notifier Status(notifier=w674) -> (notifier out=w673:refnum<notifier>, current notification=w675:T9)  [unwired: 1 in, 3 out]
              n530 = Bundle By Name(cluster=w675, "Camera Running?"=FALSE) -> (w677:T9)
              n531 = Send Notification(notification=w677, notifier=w673) -> ()  [unwired: 1 in, 2 out]
            }
            frame "Camera Soft Trigger" {
              n532 = Get Notifier Status(notifier=w758) -> (notifier out=w764:refnum<notifier>, current notification=w755:T12)  [unwired: 1 in, 3 out]
              n533 = Unbundle By Name(w755) -> ("Save Path"=w760:path, "Frames"=w739:u32, "Amp step size"=w736:dbl)
              n534 = Unbundle By Name(w733) -> ("Current Cycle"=w744:u16, "Current Step"=w743:u16, "Current Mirror Mode"=w737:u16, "Current Step"=w730:u16)
              n535 = property on="Current Laser" class="Ring (strict)"() -> ("RingText.Text"=w742:string)  [unwired: 2 in, 2 out]
              n536 = Equal To 0?(x=w730) -> (x = 0?=w729:bool)
              n537 = call "4Pi Capture File Name Increment.vi"("Path In"=w760, "Laser Line"=w742, "Cycle"=w744, "Step"=w743, "Mirror Mode"=w737, "Amp step"=u16 0, "add DM"=TRUE) -> ("Path Out"=w761:path)  [unwired: 8 in]
              n538 = Get Notifier Status(notifier=w750) -> (notifier out=w754:refnum<notifier>, current notification=w753:T9)  [unwired: 1 in, 3 out]
              n539 = Bundle By Name(cluster=w753, "Camera Running?"=TRUE) -> (w751:T9)
              n540 = call "Orca Flash Messanger.vi"("Notifier Name"=w757, "Camera Actions"=Orca_Flash_Actions."Record Settings", "Path"=w761, "# of frames"=w739) -> ("Notifier Name Dup"=w763:string)  [unwired: 7 in, 4 out]
              n541 = local read "Mirror Mode"() -> (w738:u16[])
              n542 = call "Orca Flash Messanger.vi"("Notifier Name"=w763, "Camera Actions"=Orca_Flash_Actions."SOFT TRIGGER") -> ("Notifier Name Dup"=w726:string, "Image Ref"=w756:T8)  [unwired: 9 in, 3 out]
              n543 = Send Notification(notification=w751, notifier=w754) -> (notifier out=w749:refnum<notifier>)  [unwired: 1 in, 1 out]
              n544 = Obtain Notifier(name (unnamed)=w726, notification data type=T34 {"Camera Actions"=enum."IDLE", "Received?"=FALSE, "Running?"=FALSE, "sCMOS Parameter"={"Value"=0.0, "Orca Flash Parameters"=0}, "sCMOS ROI"={"H Offset"=0, "V Offset"=0, "H Width"=0, "V Width"=0}, "Save Path"=path "", "# of frames"=0, "Image Ref"=refnum, "Trigger?"=FALSE, "bead collection"=FALSE} ("Camera Cluster")) -> (notifier out=w725:refnum<notifier>)  [unwired: 2 in, 2 out]
              n545 = while {
                tunnel: w764 -> [w789]
                tunnel: w756 -> [w785]
                tunnel: w749 -> [w773]
                tunnel: w739 -> [w783]
                tunnel: w738 -> [w788]
                tunnel: w737 -> [w787]
                tunnel: w736 -> [w786]
                tunnel: [w776] -> w735
                tunnel: [w775] -> w734
                tunnel: [w773] -> w731
                tunnel: w729 -> [w769]
                tunnel: [w768] -> w728
                tunnel: w725 -> [w766]
                i -> [w771]
                stop <- w781 stop-if-true
                n546 = Get Notifier Status(notifier=w789) -> (current notification=w791:T12)  [unwired: 1 in, 4 out]
                n547 = To Unsigned Long Integer(number=w771) -> (unsigned 32bit integer=w770:u32)
                n548 = Unbundle By Name(w791) -> ("Running?"=w780:bool)
                n549 = Increment(x=w770) -> (x+1=w772:u32)
                n550 = Greater Or Equal?(x=w772, y=w783) -> (x >= y?=w782:bool)
                n551 = flat-sequence {
                  tunnel: w783 -> [w800]
                  tunnel: w788 -> [w799]
                  tunnel: w787 -> [w798]
                  tunnel: w770 -> [w797]
                  tunnel: w786 -> [w796]
                  tunnel: w785 -> [w795]
                  tunnel: [w795] -> w784
                  tunnel: [w794] -> w774
                  tunnel: w770 -> [w794]
                  tunnel: w769 -> [w793]
                  tunnel: [w792] -> w767
                  tunnel: w766 -> [w792]
                  tunnel: w784 -> [w810]
                  tunnel: [w804] -> w775
                  tunnel: w774 -> [w803]
                  tunnel: [w802] -> w768
                  tunnel: w767 -> [w801]
                  frame #0 {
                    n552 = call "4Pi Capture Write DM.vi"("Next mode?"=w793, "Amp step size"=w796, "Current Amp Step"=w797, "Current Mirror Mode"=w798, "Mirror Mode"=w799, "No. Amp steps"=w800) -> ()  [unwired: 6 in]
                  }
                  frame #1 {
                    n553 = Get Notifier Status(notifier=w801) -> (notifier out=w809:refnum<notifier>, current notification=w808:T34)  [unwired: 1 in, 3 out]
                    n554 = Bundle By Name(cluster=w808, "Trigger?"=TRUE) -> (w806:T34)
                    n555 = Send Notification(notification=w806, notifier=w809) -> (notifier out=w802:refnum<notifier>, error out=w805:errorcluster)  [unwired: 1 in]
                    n556 = while {
                      tunnel: w810 -> [w822]
                      tunnel: w805 -> [w821]
                      tunnel: [w820] -> w804
                      tunnel: w803 -> [w818]
                      i -> [w812]
                      stop <- w811 stop-if-true
                      n557 = call "IMAQ Read Custom Data"("error in (no error)"=w821, "Key"="Image Data", "Image"=w822) -> ("Custom Data Out"=w824:string)  [unwired: 6 in, 2 out]
                      n558 = Unflatten From JSON(JSON string=w824, type and defaults=T33 {"Frame"=0, "Sensor Height"=0, "Sensor Width"=0, "ROI Height"=0, "ROI Width"=0, "ROI Enable?"=FALSE, "Bit per Pixel"=0} ("Camera IMAQ Key Info")) -> (value=w823:T33)  [unwired: 5 in, 1 out]
                      n559 = Unbundle By Name(w823) -> ("Frame"=w817:u32)
                      n560 = Wait (ms)(milliseconds to wait=u32 1) -> ()  [unwired: 1 out]
                      n561 = Greater Or Equal?(x=w812, y=1000) -> (x >= y?=w813:bool)
                      n562 = Decrement(x=w817) -> (x-1=w820:u32)
                      n563 = local write "Current Frame"(w817) -> ()
                      n564 = local write "Frame"(w817) -> ()
                      n565 = Equal?(x=w820, y=w818) -> (x = y?=w814:bool)
                      n566 = Or(x=w814, y=w813) -> (x .or. y?=w811:bool)
                    }
                  }
                }
                n567 = Not(x=w780) -> (.not. x?=w779:bool)
                n568 = Or(x=w779, y=w782) -> (x .or. y?=w781:bool)
                n569 = Wait (ms)(milliseconds to wait=u32 10) -> ()  [unwired: 1 out]
                n570 = Select(t=4Pi_Capture_Actions."Abort" ("f"), s=w779, f=4Pi_Capture_Actions."Switch") -> (s? t:f=w776:T13)
              }
              n571 = Release Notifier(notifier=w728) -> ()  [unwired: 2 in, 3 out]
              n572 = Get Notifier Status(notifier=w731) -> (notifier out=w745:refnum<notifier>, current notification=w746:T9)  [unwired: 1 in, 3 out]
              n573 = Bundle By Name(cluster=w746, "Camera Running?"=FALSE) -> (w748:T9)
              n574 = Bundle By Name(cluster=w733, "Current Amp step"=w734) -> (w732:T24)
              n575 = Send Notification(notification=w748, notifier=w745) -> ()  [unwired: 1 in, 2 out]
            }
            frame "Switch" {
              n576 = Get Notifier Status(notifier=w835) -> (current notification=w834:T12)  [unwired: 1 in, 4 out]
              n577 = Unbundle By Name(w834) -> ("Cycles"=w831:u16, "No. of Z Steps"=w832:u16)
              n578 = Bundle By Name(cluster=w833, "# of Cycles"=w831, "# of Steps"=w832) -> (w826:T24)
              n579 = Unbundle By Name(w826) -> ("Current Cycle"=w844:u16, "# of Cycles"=w843:u16, "Current Step"=w842:u16, "# of Steps"=w841:u16)
              n580 = Increment(x=w844) -> (x+1=w828:u16)
              n581 = Increment(x=w842) -> (x+1=w827:u16)
              n582 = To Single Precision Float(number=w828) -> (single precision float=w840:sgl)
              n583 = To Single Precision Float(number=w843) -> (single precision float=w839:sgl)
              n584 = To Single Precision Float(number=w827) -> (single precision float=w838:sgl)
              n585 = To Single Precision Float(number=w841) -> (single precision float=w837:sgl)
              n586 = Divide(x=w840, y=w839) -> (x/y=→"Cycle":sgl)
              n587 = Divide(x=w838, y=w837) -> (x/y=→"Z Step":sgl)
              n588 = call "4Pi Capture Scan Counter.vi"("Scan Tracker"=w826) -> ("Scan Tracker Out"=w854:T24, "Move stage?"=w847:bool, "F_MVR/T_MOV"=w851:bool, "Exit?"=w853:bool)  [unwired: 7 in]
              n589 = Select(t=4Pi_Capture_Actions."Cycle" ("y"), s=w851, f=4Pi_Capture_Actions."Step") -> (s? t:f=w848:T13)
              n590 = Select(t=w848, s=w847, f=4Pi_Capture_Actions."Setup") -> (s? t:f=w845:T13)
              n591 = Select(t=4Pi_Capture_Actions."Abort" ("y"), s=w853, f=w845) -> (s? t:f=w829:T13)
              n592 = case shown="\"Cycle\"" w829 {
                tunnel: w828 -> [_ w857 _]
                tunnel: w827 -> [_ _ w859]
                frame Default {
                }
                frame "Cycle" {
                  n593 = Increment(x=w857) -> (x+1=→"Current Cycle":u16)
                }
                frame "Step" {
                  n594 = Increment(x=w859) -> (x+1=→"Current Step":u16)
                }
              }
            }
            frame "Swtich1" {
              n595 = Unbundle By Name(w868) -> ("Current Cycle"=w880:u16, "# of Cycles"=w879:u16, "Current Step"=w878:u16, "# of Steps"=w877:u16)
              n596 = Increment(x=w880) -> (x+1=w872:u16)
              n597 = Increment(x=w878) -> (x+1=w871:u16)
              n598 = To Single Precision Float(number=w872) -> (single precision float=w876:sgl)
              n599 = To Single Precision Float(number=w879) -> (single precision float=w875:sgl)
              n600 = To Single Precision Float(number=w871) -> (single precision float=w874:sgl)
              n601 = To Single Precision Float(number=w877) -> (single precision float=w873:sgl)
              n602 = Divide(x=w876, y=w875) -> (x/y=w870:sgl)
              n603 = Divide(x=w874, y=w873) -> (x/y=w869:sgl)
              n604 = local write "Z Step"(w869) -> ()
              n605 = local write "Cycle"(w870) -> ()
              n606 = call "4Pi Capture Scan Counter 1.vi"("Scan Tracker"=w868) -> ("Scan Tracker Out"=w867:T24, "To cycle?"=w864:bool, "Move stage?"=w865:bool, "Exit?"=w866:bool)  [unwired: 7 in]
              n607 = Select(t=4Pi_Capture_Actions."Step" ("y"), s=w865, f=4Pi_Capture_Actions."Write DM") -> (s? t:f=w863:T13)
              n608 = Select(t=4Pi_Capture_Actions."Cycle" ("f"), s=w864, f=w863) -> (s? t:f=w881:T13)
              n609 = Select(t=4Pi_Capture_Actions."Abort" ("y"), s=w866, f=w881) -> (s? t:f=w861:T13)
              n610 = case shown="\"Cycle\"" w861 {
                tunnel: w872 -> [_ w886 _]
                tunnel: w871 -> [_ _ w888]
                frame Default {
                }
                frame "Cycle" {
                  n611 = Increment(x=w886) -> (x+1=w885:u16)
                  n612 = local write "Current Cycle"(w885) -> ()
                }
                frame "Step" {
                  n613 = Increment(x=w888) -> (x+1=w887:u16)
                  n614 = local write "Current Cycle"(w887) -> ()
                }
              }
            }
            frame "Step" {
              n615 = Get Notifier Status(notifier=w903) -> (current notification=w902:T12)  [unwired: 1 in, 4 out]
              n616 = Unbundle By Name(w902) -> ("Metadata File Ref"=w893:refnum<file>[], "Z Step Size (µm)"=w895:dbl, "No. of Z Steps"=w898:u16)
              n617 = Less?(x=w898, y=u16 2) -> (x < y?=w897:bool)
              n618 = Equal To 0?(x=w895) -> (x = 0?=w900:bool)
              n619 = Or(x=w900, y=w897) -> (x .or. y?=w899:bool)
              n620 = case shown="False" w899 {
                tunnel: w901 -> [w935 _]
                tunnel: w895 -> [w934 _]
                tunnel: w894 -> [w921 _]
                tunnel: w893 -> [w907 _]
                frame False {
                  # "Force the wait to happen before the position is read."
                  n621 = Unbundle By Name(w921) -> ("Current Step"=w920:u16)
                  n622 = Index Array(array=w907, index=0) -> (element=w905:refnum<file>)
                  n623 = Obtain Notifier(name (unnamed)="WFDC External Sync", notification data type=T26 {"Cycle Sync"=enum."Pause Requested", "Z Offset"=0.0, "WFDC Status"=enum."Idle"} ("WFDC External Sync"), create if not found? (T)=FALSE) -> (notifier out=w927:refnum<notifier>, error out=w933:errorcluster)  [unwired: 1 in, 1 out]
                  n624 = Get Notifier Status(notifier=w927, error in (no error)=w933) -> (notifier out=w922:refnum<notifier>, current notification=w919:T26, error out=w932:errorcluster)  [unwired: 2 out]
                  n625 = Unbundle By Name(w919) -> ("WFDC Status"=w928:T25)
                  n626 = Unbundle By Name(w932) -> ("status"=w931:bool)
                  n627 = Not Equal?(x=WFDC_Status."DC Active", y=w928) -> (x != y?=w930:bool)
                  n628 = Or(x=w930, y=w931) -> (x .or. y?=w923:bool)
                  n629 = case shown="True" w923 {
                    tunnel: w935 -> [w940 w957]
                    tunnel: w934 -> [w947 w956]
                    tunnel: w922 -> [w944 _]
                    tunnel: w920 -> [w949 _]
                    tunnel: w919 -> [w948 _]
                    tunnel: [u32 350 ("milliseconds to wait") u32 10 ("milliseconds to wait")] -> w918
                    tunnel: [w940 w950] -> w914
                    frame False {
                      n630 = To Double Precision Float(number=w949) -> (double precision float=w946:dbl)
                      n631 = Multiply(x=w947, y=w946) -> (x*y=w945:dbl)
                      n632 = Bundle By Name(cluster=w948, "Z Offset"=w945) -> (w943:T26)
                      n633 = Send Notification(notification=w943, notifier=w944) -> (notifier out=w941:refnum<notifier>)  [unwired: 1 in, 1 out]
                      n634 = Release Notifier(notifier=w941) -> ()  [unwired: 2 in, 3 out]
                    }
                    frame True {
                      n635 = Build Array(w956) -> (w955:dbl[])
                      n636 = call "Stages Messenger.vi"("Stage Notifier Name"=w957, "Actions"=Stage_Actions."MVR", "Setpoint"=w955, "Axis"=bool[] [TRUE], "Exit While Busy?"=FALSE) -> ("Stage Notifier Name (Dup)"=w950:string)  [unwired: 6 in, 4 out]
                    }
                  }
                  n637 = Wait (ms)(milliseconds to wait=w918) -> (millisecond timer value=w908:u32)
                  n638 = Set File Position(offset (in bytes) (0)=i64 0, refnum=w905, from (0:start)=enum16{"start", "end", "current"}."end") -> (refnum out=w911:refnum<file>, error out=w909:errorcluster)  [unwired: 1 in]
                  n639 = call "Stages Messenger.vi"("Stage Notifier Name"=w914, "Actions"=Stage_Actions."Get Position", "Velocity"=w908) -> ("Positions"=w916:dbl[])  [unwired: 8 in, 4 out]
                  n640 = Index Array(array=w916, index=0) -> (element=w910:dbl)
                  n641 = case shown="No Error" w909 {
                    tunnel: w911 -> [w937 _]
                    tunnel: w910 -> [w936 _]
                    frame No Error {
                      n642 = Format Value(format string="%.4f\\n", value (0)=w936) -> (output string=w939:string)  [unwired: 1 in]
                      n643 = Write to Text File(file (use dialog)=w937, text=w939) -> ()  [unwired: 2 in, 3 out]
                    }
                    frame Error {
                    }
                  }
                }
                frame True {
                }
              }
              n644 = local read "DM first"() -> (w892:bool)
              n645 = Select(t=4Pi_Capture_Actions."Write DM", s=w892, f=4Pi_Capture_Actions."Setup" ("y")) -> (s? t:f=w889:T13)
            }
            frame "Cycle" {
              w968 = T5 0 items=["Idle", "Orthogonal", "Random"] ("y")
              n646 = Unbundle By Name(w971) -> ("Current Cycle"=w970:u16)
              n647 = Get Notifier Status(notifier=w984) -> (current notification=w960:T12)  [unwired: 1 in, 4 out]
              n648 = Get Notifier Status(notifier=w975) -> (notifier out=w974:refnum<notifier>, current notification=w973:T9)  [unwired: 1 in, 3 out]
              n649 = Bundle By Name(cluster=w973, "Cycle Number"=w970) -> (w972:T9)
              n650 = Send Notification(notification=w972, notifier=w974) -> ()  [unwired: 1 in, 2 out]
              n651 = Unbundle By Name(w960) -> ("Init Z Position (µm)"=w976:dbl, "Z Step Size (µm)"=w980:dbl, "No. of Z Steps"=w979:u16)
              n652 = Unbundle By Name(w960) -> ("Sampling Time (s)"=w958:dbl)
              n653 = Equal To 0?(x=w980) -> (x = 0?=w983:bool)
              n654 = Less?(x=w979, y=u16 2) -> (x < y?=w982:bool)
              n655 = Or(x=w983, y=w982) -> (x .or. y?=w978:bool)
              n656 = Equal To 0?(x=w958) -> (x = 0?=w959:bool)
              n657 = case shown="False" w978 {
                tunnel: w977 -> [w990 _]
                tunnel: w976 -> [w992 _]
                frame False {
                  n658 = Obtain Notifier(name (unnamed)="WFDC External Sync", notification data type=T26 {"Cycle Sync"=enum."Pause Requested", "Z Offset"=0.0, "WFDC Status"=enum."Idle"} ("WFDC External Sync"), create if not found? (T)=FALSE) -> (notifier out=w998:refnum<notifier>, error out=w1004:errorcluster)  [unwired: 1 in, 1 out]
                  n659 = Get Notifier Status(notifier=w998, error in (no error)=w1004) -> (notifier out=w993:refnum<notifier>, current notification=w991:T26, error out=w1003:errorcluster)  [unwired: 2 out]
                  n660 = Unbundle By Name(w991) -> ("WFDC Status"=w999:T25)
                  n661 = Unbundle By Name(w1003) -> ("status"=w1002:bool)
                  n662 = Not Equal?(x=WFDC_Status."DC Active", y=w999) -> (x != y?=w1001:bool)
                  n663 = Or(x=w1001, y=w1002) -> (x .or. y?=w994:bool)
                  n664 = case shown="True" w994 {
                    tunnel: w993 -> [w1008 _]
                    tunnel: w992 -> [_ w1013]
                    tunnel: w991 -> [w1007 _]
                    tunnel: w990 -> [_ w1012]
                    tunnel: [u32 350 ("milliseconds to wait") u32 20 ("milliseconds to wait")] -> w989
                    frame False {
                      n665 = Bundle By Name(cluster=w1007, "Z Offset"=0.0) -> (w1010:T26)
                      n666 = Send Notification(notification=w1010, notifier=w1008) -> (notifier out=w1009:refnum<notifier>)  [unwired: 1 in, 1 out]
                      n667 = Release Notifier(notifier=w1009) -> ()  [unwired: 2 in, 3 out]
                    }
                    frame True {
                      n668 = Build Array(w1013) -> (w1014:dbl[])
                      n669 = call "Stages Messenger.vi"("Stage Notifier Name"=w1012, "Actions"=Stage_Actions."MOVE", "Setpoint"=w1014, "Axis"=bool[] [TRUE], "Exit While Busy?"=FALSE) -> ()  [unwired: 6 in, 5 out]
                    }
                  }
                  n670 = Wait (ms)(milliseconds to wait=w989) -> ()  [unwired: 1 out]
                }
                frame True {
                }
              }
              n671 = case shown="False" w959 {
                tunnel: w958 -> [w988 _]
                frame False {
                  n672 = Multiply(x=w988, y=1000.0) -> (x*y=w986:dbl)
                  n673 = Wait (ms)(milliseconds to wait=w986) -> ()  [unwired: 1 out]
                }
                frame True {
                }
              }
              n674 = local read "Soft trigger"() -> (w961:bool)
              n675 = local read "DM scan mode"() -> (w965:T5)
              n676 = Select(t=4Pi_Capture_Actions."External Cycle Sync" ("f"), s=w961, f=4Pi_Capture_Actions."Write DM") -> (s? t:f=w962:T13)
              n677 = Equal?(x=w965, y=w968) -> (x = y?=w967:bool)
              n678 = Select(t=4Pi_Capture_Actions."External Cycle Sync" ("y"), s=w967, f=w962) -> (s? t:f=w966:T13)
            }
            frame "Write DM" {
              n679 = Get Notifier Status(notifier=w1035) -> (current notification=w1034:T12)  [unwired: 1 in, 4 out]
              n680 = Unbundle By Name(w1026) -> ("Current Mirror Mode"=w1031:u16, "Current Amp step"=w1032:u16, "Current Step"=w1018:u16)
              n681 = Unbundle By Name(w1034) -> ("DM scan mode"=w1028:T5, "Amp step size"=w1030:dbl, "No. Amp steps"=w1029:u16, "Metadata File Ref"=w1027:refnum<file>[])
              n682 = local read "Mirror Mode"() -> (w1033:u16[])
              n683 = case shown="1, Default" w1028 {
                tunnel: [w1038 w1095] -> w1037
                tunnel: w1033 -> [w1043 w1091]
                tunnel: w1032 -> [_ w1078]
                tunnel: w1031 -> [_ w1076]
                tunnel: w1030 -> [_ w1083]
                tunnel: w1029 -> [_ w1082]
                tunnel: w1027 -> [w1042 _]
                tunnel: w1018 -> [_ w1071]
                frame 2 {
                  w1044 = 4Pi_Dual_DM_-_Standard_Action."Read" ("Action")
                  n684 = Index Array(array=w1042, index=1) -> (element=w1040:refnum<file>)
                  n685 = Refnum to Path(1:w1040) -> (0:w1039:path)
                  n686 = call "4Pi Dual DM - Mirror Mode DUAL AE.vi"("Action"=w1044) -> ("Mirror Modes Out"=w1051:T36)  [unwired: 14 in]
                  n687 = call "4Pi Dual DM - Active Mirror AE.vi"("Action"=w1044) -> ("Active Mirror"=w1052:i32)  [unwired: 14 in]
                  n688 = Initialize Array(0.0 ("element"), 0 ("dimension size")) -> (w1048:dbl[])
                  n689 = Index Array(array=w1051, index (col)=w1052) -> (element=w1045:cluster{"Mode":string, "Amplitude":dbl}[])  [unwired: 1 in]
                  n690 = for {
                    tunnel: w1043 -> [w1058] mode=indexing
                    shift-right: [w1065] -> w1055
                    shift-left: w1048 -> [w1066]
                    tunnel: "Amp magnitude" -> [w1063]
                    shift-right: [w1060] -> w1050
                    shift-left: w1045 -> [w1061]
                    n691 = Decrement(x=w1058) -> (x-1=w1057:u16)
                    n692 = Multiply(x=w1063, y=2.0) -> (x*y=w1070:dbl)
                    n693 = Random Number (0-1)() -> (number: 0 to 1=w1068:dbl)
                    n694 = Multiply(x=w1068, y=w1070) -> (x*y=w1067:dbl)
                    n695 = Index Array(array=w1061, index=w1057) -> (element=w1064:cluster{"Mode":string, "Amplitude":dbl})
                    n696 = Subtract(x=w1067, y=w1063) -> (x-y=w1062:dbl)
                    n697 = Bundle By Name(cluster=w1064, "Amplitude"=w1062) -> (w1059:cluster{"Mode":string, "Amplitude":dbl})
                    n698 = Build Array (concatenate)(w1066, w1062) -> (w1065:dbl[])
                    n699 = Replace Array Subset(array=w1061, new element=w1059, index=w1057) -> (w1060:cluster{"Mode":string, "Amplitude":dbl}[])
                  }
                  n700 = Replace Array Subset(array=w1051, new element=w1050, index (col)=w1052) -> (w1038:T36)  [unwired: 1 in]
                  n701 = call-poly <vilib>:"Write Delimited Spreadsheet.vi"("file path (dialog if empty)"=w1039, "format (%.3f)"="%.4f", "1D data"=w1055, "append to file? (new file:F)"=TRUE, "delimiter (\\t)"="," ("delimiter (\\t)")) -> ()  [unwired: 9 in, 2 out]
                }
                frame 1, Default {
                  w1097 = 4Pi_Dual_DM_-_Standard_Action."Read" ("Action")
                  n702 = Equal To 0?(x=w1076) -> (x = 0?=w1077:bool)
                  n703 = Decrement(x=w1082) -> (x-1=w1081:u16)
                  n704 = case shown="True" w1077 {
                    tunnel: [w1099 w1100] -> w1090
                    tunnel: w1076 -> [w1098 w1100]
                    frame False {
                      n705 = Decrement(x=w1098) -> (x-1=w1099:u16)
                    }
                    frame True {
                    }
                  }
                  n706 = To Double Precision Float(number=w1081) -> (double precision float=w1080:dbl)
                  n707 = call "4Pi Dual DM - Mirror Mode DUAL AE.vi"("Action"=w1097) -> ("Mirror Modes Out"=w1096:T36)  [unwired: 14 in]
                  n708 = call "4Pi Dual DM - Active Mirror AE.vi"("Action"=w1097) -> ("Active Mirror"=w1092:i32)  [unwired: 14 in]
                  n709 = Divide(x=w1080, y=2.0) -> (x/y=w1085:dbl)
                  n710 = Index Array(array=w1091, index #1=w1090, index #2=w1076) -> (element #1=w1074:u16, element #2=w1073:u16)
                  n711 = Index Array(array=w1096, index (col)=w1092) -> (element=w1093:cluster{"Mode":string, "Amplitude":dbl}[])  [unwired: 1 in]
                  n712 = Multiply(x=w1083, y=w1085) -> (x*y=w1079:dbl)
                  n713 = Decrement(x=w1074) -> (x-1=w1075:u16)
                  n714 = Decrement(x=w1073) -> (x-1=w1072:u16)
                  n715 = Index Array(array=w1093, index #1=w1075, index #2=w1072) -> (element #1=w1088:cluster{"Mode":string, "Amplitude":dbl}, element #2=w1089:cluster{"Mode":string, "Amplitude":dbl})
                  n716 = case shown="0" w1078 {
                    tunnel: w1089 -> [w1114 w1126]
                    tunnel: w1083 -> [_ w1124]
                    tunnel: [w1112 w1122] -> w1086
                    tunnel: w1088 -> [w1110 w1121]
                    tunnel: [w1108 w1121] -> w1087
                    tunnel: w1079 -> [w1103 _]
                    tunnel: w1071 -> [w1107 _]
                    frame 0 {
                      n717 = Not Equal To 0?(x=w1107) -> (x != 0?=w1105:bool)
                      n718 = local read "DM first"() -> (w1106:bool)
                      n719 = Unbundle By Name(w1110) -> ("Amplitude"=w1111:dbl)
                      n720 = Unbundle By Name(w1114) -> ("Amplitude"=w1115:dbl)
                      n721 = Compound Arithmetic op=AND(w1106, w1105) -> (w1104:bool)
                      n722 = case shown="True" w1104 {
                        tunnel: w1103 -> [w1116 w1120]
                        tunnel: [w1116 w1118] -> w1102
                        tunnel: [w1116 0.0] -> w1101
                        frame False {
                        }
                        frame True {
                          n723 = Multiply(x=w1120, y=2.0) -> (x*y=w1118:dbl)
                        }
                      }
                      n724 = Subtract(x=w1111, y=w1101) -> (x-y=w1109:dbl)
                      n725 = Subtract(x=w1115, y=w1102) -> (x-y=w1113:dbl)
                      n726 = Bundle By Name(cluster=w1110, "Amplitude"=w1109) -> (w1108:cluster{"Mode":string, "Amplitude":dbl})
                      n727 = Bundle By Name(cluster=w1114, "Amplitude"=w1113) -> (w1112:cluster{"Mode":string, "Amplitude":dbl})
                    }
                    frame Default {
                      n728 = Unbundle By Name(w1126) -> ("Amplitude"=w1125:dbl)
                      n729 = Add(x=w1125, y=w1124) -> (x+y=w1123:dbl)
                      n730 = Bundle By Name(cluster=w1126, "Amplitude"=w1123) -> (w1122:cluster{"Mode":string, "Amplitude":dbl})
                    }
                  }
                  n731 = Replace Array Subset(array=w1093, new element #1=w1087, index #1=w1075, new element #2=w1086, index #2=w1072) -> (w1094:cluster{"Mode":string, "Amplitude":dbl}[])
                  n732 = Replace Array Subset(array=w1096, new element=w1094, index (col)=w1092) -> (w1095:T36)  [unwired: 1 in]
                }
              }
              n733 = Unbundle By Name(w1026) -> ("Current Amp step"=w1025:u16)
              n734 = flat-sequence {
                tunnel: w1037 -> [w1127]
                frame #0 {
                  n735 = call "4Pi Dual DM - Mirror Mode DUAL AE.vi"("Action"=4Pi_Dual_DM_-_Standard_Action."Write", "Mirror Modes In"=w1127) -> ()  [unwired: 13 in, 1 out]
                }
                frame #1 {
                  w1129 = "Mirror Control Que" ("name (unnamed)")
                  n736 = Obtain Queue(max queue size (-1, unlimited)=10, name (unnamed)=w1129, element data type=w1129, create if not found? (T)=FALSE) -> (queue out=w1133:refnum<queue>, error out=w1132:errorcluster)  [unwired: 1 in, 1 out]
                  n737 = case shown="No Error" w1132 {
                    tunnel: w1133 -> [w1134 _]
                    frame No Error {
                      n738 = Enqueue Element(queue=w1134, element="Mirror Modes" ("name (unnamed)")) -> ()  [unwired: 2 in, 3 out]
                    }
                    frame Error {
                      n739 = One Button Dialog(message="DMs not found.") -> ()  [unwired: 1 in, 1 out]
                    }
                  }
                }
              }
              n740 = local read "DM first"() -> (w1024:bool)
              n741 = Not Equal To 0?(x=w1025) -> (x != 0?=w1023:bool)
              n742 = Compound Arithmetic op=AND(w1024, w1023) -> (w1022:bool)
              n743 = Select(t=4Pi_Capture_Actions."Setup", s=w1022, f=4Pi_Capture_Actions."External Cycle Sync" ("y")) -> (s? t:f=w1019:T13)
            }
            frame "External Cycle Sync" {
              n744 = Obtain Notifier(name (unnamed)="WFDC External Sync", notification data type=T26 {"Cycle Sync"=enum."Pause Requested", "Z Offset"=0.0, "WFDC Status"=enum."Idle"} ("WFDC External Sync"), create if not found? (T)=FALSE) -> (notifier out=w1155:refnum<notifier>, error out=w1158:errorcluster)  [unwired: 1 in, 1 out]
              n745 = Get Notifier Status(notifier=w1155, error in (no error)=w1158) -> (notifier out=w1144:refnum<notifier>, current notification=w1143:T26, error out=w1157:errorcluster)  [unwired: 2 out]
              n746 = Unbundle By Name(w1157) -> ("status"=w1151:bool)
              n747 = Unbundle By Name(w1143) -> ("WFDC Status"=w1142:T25, "Cycle Sync"=w1150:T27)
              n748 = Not(x=w1151) -> (.not. x?=w1146:bool)
              n749 = Equal?(x=WFDC_Status."Error", y=w1142) -> (x = y?=w1140:bool)
              n750 = Equal?(x=WFDC_Status."DC Active", y=w1142) -> (x = y?=w1148:bool)
              n751 = Equal?(x=w1150, y=WFDC_Cycle_Pause."Pause Requested") -> (x = y?=w1147:bool)
              n752 = Compound Arithmetic op=AND(w1148, w1147, w1146) -> (w1145:bool)
              n753 = case shown="True" w1145 {
                tunnel: w1144 -> [_ w1168]
                tunnel: w1143 -> [_ w1170]
                frame False {
                }
                frame True {
                  n754 = Bundle By Name(cluster=w1170, "Cycle Sync"=WFDC_Cycle_Pause."Paused") -> (w1167:T26)
                  n755 = Send Notification(notification=w1167, notifier=w1168) -> (notifier out=w1166:refnum<notifier>)  [unwired: 1 in, 1 out]
                  n756 = while {
                    tunnel: w1166 -> [w1181]
                    tunnel: [w1172] -> w1163
                    tunnel: [w1171] -> w1165
                    i -> [w1177]
                    stop <- w1173 stop-if-true
                    n757 = Get Notifier Status(notifier=w1181) -> (notifier out=w1172:refnum<notifier>, current notification=w1171:T26)  [unwired: 1 in, 3 out]
                    n758 = Greater?(x=w1177, y=15000) -> (0:w1174:bool)
                    n759 = Unbundle By Name(w1171) -> ("Cycle Sync"=w1180:T27)
                    n760 = Equal?(x=w1180, y=WFDC_Cycle_Pause."Resume Requested") -> (x = y?=w1175:bool)
                    n761 = Or(x=w1175, y=w1174) -> (x .or. y?=w1173:bool)
                    n762 = Wait (ms)(milliseconds to wait=u32 1) -> ()  [unwired: 1 out]
                  }
                  n763 = Bundle By Name(cluster=w1165, "Cycle Sync"=WFDC_Cycle_Pause."Resumed") -> (w1162:T26)
                  n764 = Send Notification(notification=w1162, notifier=w1163) -> (notifier out=w1161:refnum<notifier>)  [unwired: 1 in, 1 out]
                  n765 = Release Notifier(notifier=w1161) -> ()  [unwired: 2 in, 3 out]
                }
              }
              n766 = Select(t=4Pi_Capture_Actions."Abort" ("y"), s=w1140, f=4Pi_Capture_Actions."Setup" ("y")) -> (s? t:f=w1138:T13)
            }
            frame "Quit" {
            }
          }
        }
      }
      n767 = local write "Quit"(w228) -> ()
      n768 = Release Notifier(notifier=w185) -> ()  [unwired: 2 in, 3 out]
    }
    frame Error {
      n769 = Release Notifier(notifier=w1624) -> (error out=w1623:errorcluster)  [unwired: 2 in, 2 out]
      n770 = for {
        tunnel: w1622 -> [w1629] mode=indexing
        n771 = call "IMAQ Dispose"("Image"=w1629) -> ()  [unwired: 5 in, 1 out]
      }
      n772 = Unbundle By Name(w1623) -> ("source"=w1626:string)
      n773 = Concatenate Strings("4Pi Capture Manager could not start.", "\r", w1626) -> (w1625:string)
      n774 = One Button Dialog(message=w1625) -> ()  [unwired: 1 in, 1 out]
    }
  }
  n775 = control-ref of="This VI"() -> (w121:refnum<vi>)
  n776 = property class="VI"(reference=w121) -> (reference out=w130:refnum<vi>, "Panel"=w122:refnum<vi>)  [unwired: 1 in, 1 out]
  n777 = property class="Pnl"(reference=w122) -> ("Decos[]"=w120:refnum<vi>[], "Panes[]"=w126:refnum<vi>[])  [unwired: 1 in, 2 out]
  n778 = Array Size(array=w120) -> (size(s)=w118:i32)
  n779 = Decrement(x=w118) -> (x-1=w119:i32)
  n780 = Index Array(array=w126, index=0) -> (element=w125:refnum<vi>)
  n781 = Index Array(array=w120, index=w119) -> (element=w128:refnum<vi>)
  n782 = property class="VI"(reference=w130) -> (reference out=w132:refnum<vi>, "Front Panel.PanelBounds"=w133:T37)  [unwired: 1 in, 1 out]
  n783 = property class="Decor"(reference=w128) -> ("Bounds"=w131:T38)  [unwired: 1 in, 2 out]
  n784 = property class="Pane"(reference=w125, "Origin"=T16 {"Horizontal"=0, "Vertical"=0}, "HorizScrollbarVisibility"=w129, "VertScrollbarVisibility"=w129) -> ()  [unwired: 1 in, 2 out]
  n785 = Unbundle By Name(w131) -> ("Width"=w136:u32, "Height"=w139:u32)
  n786 = control-ref of="Quit"() -> (w123:refnum<vi>)
  n787 = To Word Integer(number=w136) -> (16bit integer=w138:i16)
  n788 = To Word Integer(number=w139) -> ()  [unwired: 1 out]
  n789 = property class="Bool (strict)"(reference=w123) -> ("Height"=w141:u32, "Top"=w142:i32)  [unwired: 1 in, 2 out]
  n790 = Unbundle By Name(w133) -> ("Left"=w135:i16, "Top"=w146:i16)
  n791 = To Word Integer(number=w141) -> (16bit integer=w144:i16)
  n792 = To Word Integer(number=w142) -> (16bit integer=w145:i16)
  n793 = Add(x=w135, y=w138) -> (x+y=w137:i16)
  n794 = Compound Arithmetic op=ADD(w146, w144, w145, i16 12 ("y")) -> (w140:i16)
  n795 = Bundle By Name(cluster=w133, "Right"=w137, "Bottom"=w140) -> (w134:T37)
  n796 = property class="VI"(reference=w132, "Front Panel.PanelBounds"=w134) -> ()  [unwired: 1 in, 2 out]
